vi "Periodic Tasks.vi"(8 "error in":errorcluster, 11 "RobotConfig":T17={"Motors"={"DriveLeftPrimary"={"CAN Address"=0, "Invert"=FALSE, "InvertSensor"=FALSE, "Unit Conversion Factor"=0.0, "Brake Mode"=enum."Override to Brake", "Reverse Limt Switch Mode"=enum."Normally Closed", "Forward Limt Swith Mode"=enum."Normally Closed", "PWM Channel"=enum."Invalid", "Motor Controller Type"=enum."Talon SRX"}, "DriveLeftSecondary1"={"CAN Address"=0, "Invert"=FALSE, "InvertSensor"=FALSE, "Unit Conversion Factor"=0.0, "Brake Mode"=enum."Override to Brake", "Reverse Limt Switch Mode"=enum."Normally Closed", "Forward Limt Swith Mode"=enum."Normally Closed", "PWM Channel"=enum."Invalid", "Motor Controller Type"=enum."Talon SRX"}, "DriveRightPrimary"={"CAN Address"=0, "Invert"=FALSE, "InvertSensor"=FALSE, "Unit Conversion Factor"=0.0, "Brake Mode"=enum."Override to Brake", "Reverse Limt Switch Mode"=enum."Normally Closed", "Forward Limt Swith Mode"=enum."Normally Closed", "PWM Channel"=enum."Invalid", "Motor Controller Type"=enum."Talon SRX"}, "DriveRightSecondary1"={"CAN Address"=0, "Invert"=FALSE, "InvertSensor"=FALSE, "Unit Conversion Factor"=0.0, "Brake Mode"=enum."Override to Brake", "Reverse Limt Switch Mode"=enum."Normally Closed", "Forward Limt Swith Mode"=enum."Normally Closed", "PWM Channel"=enum."Invalid", "Motor Controller Type"=enum."Talon SRX"}, "RightIntake"={"CAN Address"=8, "Invert"=FALSE, "InvertSensor"=FALSE, "Unit Conversion Factor"=0.0, "Brake Mode"=enum."Override to Brake", "Reverse Limt Switch Mode"=enum."Normally Closed", "Forward Limt Swith Mode"=enum."Normally Closed", "PWM Channel"=enum."Invalid", "Motor Controller Type"=enum."Talon SRX"}, "LeftIntake"={"CAN Address"=7, "Invert"=FALSE, "InvertSensor"=FALSE, "Unit Conversion Factor"=0.0, "Brake Mode"=enum."Override to Brake", "Reverse Limt Switch Mode"=enum."Normally Closed", "Forward Limt Swith Mode"=enum."Normally Closed", "PWM Channel"=enum."Invalid", "Motor Controller Type"=enum."Talon SRX"}, "ArmPivot"={"CAN Address"=5, "Invert"=FALSE, "InvertSensor"=FALSE, "Unit Conversion Factor"=0.0, "Brake Mode"=enum."Override to Brake", "Reverse Limt Switch Mode"=enum."Normally Closed", "Forward Limt Swith Mode"=enum."Normally Closed", "PWM Channel"=enum."Invalid", "Motor Controller Type"=enum."Talon SRX"}, "ArmExtend"={"CAN Address"=6, "Invert"=FALSE, "InvertSensor"=FALSE, "Unit Conversion Factor"=0.0, "Brake Mode"=enum."Override to Brake", "Reverse Limt Switch Mode"=enum."Normally Closed", "Forward Limt Swith Mode"=enum."Normally Closed", "PWM Channel"=enum."Invalid", "Motor Controller Type"=enum."Talon SRX"}, "ArmPivot2"={"CAN Address"=9, "Invert"=FALSE, "InvertSensor"=FALSE, "Unit Conversion Factor"=0.0, "Brake Mode"=enum."Override to Brake", "Reverse Limt Switch Mode"=enum."Normally Closed", "Forward Limt Swith Mode"=enum."Normally Closed", "PWM Channel"=enum."Invalid", "Motor Controller Type"=enum."Talon SRX"}, "Climber"={"CAN Address"=10, "Invert"=FALSE, "InvertSensor"=FALSE, "Unit Conversion Factor"=0.0, "Brake Mode"=enum."Override to Brake", "Reverse Limt Switch Mode"=enum."Disabled", "Forward Limt Swith Mode"=enum."Disabled", "PWM Channel"=enum."Invalid", "Motor Controller Type"=enum."Talon SRX"}, "Selfie Stick"={"CAN Address"=11, "Invert"=FALSE, "InvertSensor"=FALSE, "Unit Conversion Factor"=0.0, "Brake Mode"=enum."Override to Brake", "Reverse Limt Switch Mode"=enum."Disabled", "Forward Limt Swith Mode"=enum."Disabled", "PWM Channel"=enum."Invalid", "Motor Controller Type"=enum."Talon SRX"}}, "Sensors"={"IMU"={"Yaw Axis"=enum."X", "SPI Bus"=enum."SPI MXP", "AHRS Algorithm"=enum."Complementary", "Calibration Time (s)"=3.0, "Calibrate On Open"=FALSE}, "LimitSwitch1"={"DIOChannel"=enum."DIO 0", "Active Low"=FALSE}, "LimitSwitch2"={"DIOChannel"=enum."DIO 1", "Active Low"=FALSE}, "BeamBreak"={"DIOChannel"=enum."DIO 2", "Active Low"=FALSE}, "JeVois"={"Baud Rate"=9600, "Parity"=0, "Data Bits"=8, "Stop Bits"=10, "Termination Char (0xA = '\\n' = LF)"=10, "Enable Termination Char? (T)"=TRUE, "Flow Control"=0, "Timeout Value (ms)"=5000, "Serial Port"=enum."Onboard RS-232"}}, "PID"={"ArmExtend"={"P"=0.0, "I"=0.0, "D"=0.0, "F"=0.0, "IZone"=0.0}, "ArmRotate"={"P"=0.0, "I"=0.0, "D"=0.0, "F"=0.0, "IZone"=0.0}, "Drive"={"P"=0.0, "I"=0.0, "D"=0.0, "F"=0.0, "IZone"=0.0}, "DriveGyro Kp ((in/sec)/deg)"=0.0, "CameraPole"={"P"=0.0, "I"=0.0, "D"=0.0, "F"=0.0, "IZone"=0.0}}, "Solenoids"={"ArmClaw"={"Forward Channel"=enum."Solenoid 0", "Invert"=FALSE, "Reverse Channel"=enum."Solenoid 0"}, "IntakeExtend"={"Forward Channel"=enum."Solenoid 1", "Invert"=FALSE, "Reverse Channel"=enum."Solenoid 0"}, "IntakeOpen"={"Forward Channel"=enum."Solenoid 2", "Invert"=FALSE, "Reverse Channel"=enum."Solenoid 0"}, " Shifter"={"Forward Channel"=enum."Solenoid 3", "Invert"=FALSE, "Reverse Channel"=enum."Solenoid 0"}}, "RobotDimensions "={"Length"=0.0, "Height"=0.0, "HeightOfBumpers"=0.0, "DistanceFromFrameEdgeToPyramid "=0.0, "HeightOfFrameToIntake"=0.0, "EdgeOfFrameToOrigin"=0.0}, "ArmHomePosition"={"Angle (rad)"=0.0, "Radius (in)"=0.0}, "SelfieStickParams"={"Home Height (in)"=0.0, "CruiseVelocity"=0, "MaxAccel"=0, "Low Height (in)"=0.0, "High Height (in)"=0.0, "Mid Height (in)"=0.0}, "Enable Compressor"=TRUE} {"Sensors"."JeVois"."Flow Control" items=["None", "XON/XOFF", "RTS/CTS", "XON/XOFF & RTS/CTS", "DTR/DSR", "XON/XOFF & DTR/DSR"]; "Sensors"."JeVois"."Termination Char (0xA = '\\n' = LF)" format="%.0x"; "Sensors"."JeVois"."Stop Bits" items=["1.0"=10, "1.5"=15, "2.0"=20]; "Sensors"."JeVois"."Parity" items=["None", "Odd", "Even", "Mark", "Space"]}) -> ()   [LabVIEW 2017]
doc: "This VI runs in parallel to other tasks. It can contain as many user-defined periodic loops as you need. These can carry out PID or other sorts of timed response."
uses:
  PowerUpSrc/TypeDefs/ConfigComponents/Config_Robot.ctl
  ArgosLib/Config/ConfigComponents/TypeDefs/Config_Motor.ctl
  <vilib>/Rock Robotics/WPI/ThirdParty/Phoenix-LabVIEW/Motor Controller/Controls/CTRE_Phoenix_MotorControl_NeutralMode.ctl
  <vilib>/Rock Robotics/WPI/ThirdParty/Phoenix-LabVIEW/Motor Controller/Controls/CTRE_Phoenix_MotorControl_LimitSwitchNormal.ctl
  <vilib>/Rock Robotics/SystemInterfaces/DIO/FPGA_DIOPWMChannel.ctl
  ArgosLib/Config/ConfigComponents/TypeDefs/Config_MotorCtrlType.ctl
  ArgosLib/Config/ConfigComponents/TypeDefs/Config_IMU.ctl
  <vilib>/Rock Robotics/SystemInterfaces/spilib/spi_bus.ctl
  ArgosLib/Config/ConfigComponents/TypeDefs/Config_DigitalIO.ctl
  <vilib>/Rock Robotics/SystemInterfaces/DIO/FPGA_DIOChannel.ctl
  ArgosLib/Config/ConfigComponents/TypeDefs/Config_SerialPort.ctl
  <vilib>/Rock Robotics/WPI/SerialPort/WPI_SerialPort.ctl
  ArgosLib/Config/ConfigComponents/TypeDefs/Config_PIDParams.ctl
  ArgosLib/Config/ConfigComponents/TypeDefs/Config_DoubleSolenoid.ctl
  <vilib>/Rock Robotics/WPI/Solenoid/WPI_SolenoidChannel.ctl
  PowerUpSrc/TypeDefs/ConfigComponents/Config_Dimensions.ctl
  PowerUpSrc/TypeDefs/ConfigComponents/Config_ArmHome.ctl
  PowerUpSrc/TypeDefs/ConfigComponents/Config_SelfieStick.ctl
  ArgosLib/Miscellaneous/TypeDefs/ArgoDriveJoystickMap.ctl
  ArgosLib/Miscellaneous/TypeDefs/LookUpTableParameters.ctl
  PowerUpSrc/Implements/Arm/TypeDefs/ArmPositions.ctl
  ArgosLib/Path Planning/TypeDefs/Point2D.ctl
  PowerUpSrc/General/MotionProfiling/TypeDefs/MotionProfileGeneratorParams.ctl
  <vilib>/Rock Robotics/WPI/ThirdParty/Phoenix-LabVIEW/Motor Controller/Controls/CTRE_Phoenix_MotorControl_TrajectoryPointTimeDur.ctl
  PowerUpSrc/Autonomous/PathPlannerSupport/TypeDefs/DrivePathfinderParams.ctl
  PowerUpSrc/Autonomous/TypeDef/AutoStep.ctl
  PowerUpSrc/Autonomous/TypeDef/AutoWaypointType.ctl
  Pathfinder/Pathfinder-LabVIEW/Pathfinder-Lib/VIs/Waypoint.ctl
  PowerUpSrc/Implements/Arm/TypeDefs/ArmTargetPosition.ctl
  PowerUpSrc/Implements/TypeDefs/IntakeState.ctl
  PowerUpSrc/Autonomous/TypeDef/AutoStartingPositions.ctl
  PowerUpSrc/Autonomous/TypeDef/AutoFieldState.ctl
  <vilib>/Rock Robotics/WPI/DriverStation/WPI_DriverStationRobotMode2.ctl
  ArgosLib/Signal Processing/TypeDefs/EdgeDetector_Type.ctl
  <vilib>/Rock Robotics/WPI/Solenoid/WPI_SolenoidValue.ctl
  PowerUpSrc/Implements/Arm/TypeDefs/ArmHomingState.ctl
  PowerUpSrc/General/MotionProfiling/TypeDefs/MotionProfileControlState.ctl
  <vilib>/Rock Robotics/WPI/ThirdParty/Phoenix-LabVIEW/Motor Controller/Controls/CTRE_Phoenix_MotorControl_ControlMode.ctl
  <vilib>/Rock Robotics/WPI/Utilities/WPI_GetSetVariantRefNum.vi
  PowerUpSrc/Global_Var-RefNum/LEDData.vi
  PowerUpSrc/Global_Var-RefNum/Joystick_Control.vi
  <vilib>/Rock Robotics/WPI/Solenoid/WPI_SolenoidSetEnum.vi
  PowerUpSrc/Global_Var-RefNum/SwitchedCameraData.vi
  ArgosLib/ArgosLib.lvlib
  PowerUpSrc/Sensors/IMU/ADIS16448_IMU.lvlib
  69abced5-d8d5-48e2-b3a2-692bc54adc8e.vi
  Pathfinder/Pathfinder-LabVIEW/Pathfinder-Lib/Pathfinder.lvlib
panel:
  out "ActiveTestRoutine":string
  in  "AutoTest":bool
  out "AutoControl":bool
  out "ArmReadyForAuto":bool
  out "LED Loop Rate (Hz)":dbl
  in  "Reload Routines":bool
  in  "Auto Routines Storage Directory":path=path "/home/lvuser/AutoRoutines"
  in  "Auto Routine":u16(ring) items=["Auto Line", "Auto Line (Reverse)", "Left Switch->Left Scale", "Left Switch->Left Switch->Left Scale", "Left Switch->Left Switch", "Left Switch->Left Switch (Back)", "Left Switch->Right Scale", "Left Switch", "Right Switch->Left Scale", "Right Switch->Right Scale", "Right Switch->Right Switch->Right Scale", "Right Switch->Right Switch", "Right Switch->Right Switch (Back)", "Right Switch"]
  in  "AutoStartingPosition":T1
  in  "CustomAutoSteps":bool
  in  "AutoInTeleop":bool
  in  "AutoStart":bool
  out "AutoIntakeState":T2
  out "AutoClawOpen":bool
  in  "AutoSteps":T3[](array[typedef])=[{"Waypoint Type"=enum."Pathfinder Endpoint", "Waypoint"={"x"=19.5, "y"=50.0, "angle"=0.0}, "WaitTime (ms)"=0, "ArmPosition"=enum."Hold", "IntakeState"=enum."Stop", "Claw Open"=FALSE, "ArmOffsetTime (ms)"=0, "ClawReleaseTime (ms)"=0}, {"Waypoint Type"=enum."Pathfinder Waypoint", "Waypoint"={"x"=180.0, "y"=50.0, "angle"=0.0}, "WaitTime (ms)"=0, "ArmPosition"=enum."Hold", "IntakeState"=enum."Stop", "Claw Open"=FALSE, "ArmOffsetTime (ms)"=0, "ClawReleaseTime (ms)"=0}, {"Waypoint Type"=enum."Pathfinder Waypoint", "Waypoint"={"x"=270.0, "y"=135.0, "angle"=90.0}, "WaitTime (ms)"=0, "ArmPosition"=enum."Hold", "IntakeState"=enum."Stop", "Claw Open"=FALSE, "ArmOffsetTime (ms)"=0, "ClawReleaseTime (ms)"=0}, {"Waypoint Type"=enum."Pathfinder Waypoint", "Waypoint"={"x"=270.0, "y"=260.0, "angle"=90.0}, "WaitTime (ms)"=0, "ArmPosition"=enum."Hold", "IntakeState"=enum."Stop", "Claw Open"=FALSE, "ArmOffsetTime (ms)"=0, "ClawReleaseTime (ms)"=0}, {"Waypoint Type"=enum."Pathfinder Endpoint", "Waypoint"={"x"=180.0, "y"=350.0, "angle"=180.0}, "WaitTime (ms)"=0, "ArmPosition"=enum."Hold", "IntakeState"=enum."Stop", "Claw Open"=FALSE, "ArmOffsetTime (ms)"=0, "ClawReleaseTime (ms)"=0}, {"Waypoint Type"=enum."Zero-Radius Turn Endpoint", "Waypoint"={"x"=0.0, "y"=0.0, "angle"=180.0}, "WaitTime (ms)"=0, "ArmPosition"=enum."Hold", "IntakeState"=enum."Stop", "Claw Open"=FALSE, "ArmOffsetTime (ms)"=0, "ClawReleaseTime (ms)"=0}, {"Waypoint Type"=enum."Zero-Radius Turn Endpoint", "Waypoint"={"x"=0.0, "y"=0.0, "angle"=290.0}, "WaitTime (ms)"=0, "ArmPosition"=enum."Switch", "IntakeState"=enum."Stop", "Claw Open"=FALSE, "ArmOffsetTime (ms)"=0, "ClawReleaseTime (ms)"=0}, {"Waypoint Type"=enum."Pathfinder Endpoint", "Waypoint"={"x"=180.0, "y"=320.0, "angle"=270.0}, "WaitTime (ms)"=0, "ArmPosition"=enum."Switch", "IntakeState"=enum."Stop", "Claw Open"=FALSE, "ArmOffsetTime (ms)"=0, "ClawReleaseTime (ms)"=0}, {"Waypoint Type"=enum."Pathfinder Endpoint", "Waypoint"={"x"=180.0, "y"=300.0, "angle"=270.0}, "WaitTime (ms)"=0, "ArmPosition"=enum."Switch", "IntakeState"=enum."Stop", "Claw Open"=FALSE, "ArmOffsetTime (ms)"=0, "ClawReleaseTime (ms)"=0}, {"Waypoint Type"=enum."Stationary", "Waypoint"={"x"=0.0, "y"=0.0, "angle"=0.0}, "WaitTime (ms)"=250, "ArmPosition"=enum."Hold", "IntakeState"=enum."Stop", "Claw Open"=TRUE, "ArmOffsetTime (ms)"=0, "ClawReleaseTime (ms)"=0}]
  out "Auto Loop Rate (Hz)":dbl
  in  "DrivePathPlanParams":T7={"max_velocity (in/s)"=70.0, "max_acceleration (in/s^2)"=200.0, "max_jerk (in/s^3)"=300.0, "dt(ms)"=40, "sample_count"=1000, "wheelbase_width (in)"=25.0} {"dt(ms)" items=["TrajectoryDuration_0ms"=0, "TrajectoryDuration_5ms"=5, "TrajectoryDuration_10ms"=10, "TrajectoryDuration_20ms"=20, "TrajectoryDuration_30ms"=30, "TrajectoryDuration_40ms"=40, "TrajectoryDuration_50ms"=50, "TrajectoryDuration_100ms"=100]}
  in  "DriveGyro Kp ((in/sec)/deg)":dbl=-0.5
  in  "Turning_Still_Multiplier":dbl=2.5
  out "IMU Angles Out":T9
  out "Drive Velocity Loop Rate (Hz)":dbl
  out "Arm Planner Loop Rate (Hz)":dbl
  out "Drive Planner Loop Rate (Hz)":dbl
  out "MP Loop Rate (Hz)":dbl
  out "Implement Loop Rate (Hz)":dbl
  out "JeVois Loop Rate (Hz)":dbl
  out "Compressor Loop Rate (Hz)":dbl
  out "Drive Loop Rate (Hz)":dbl
  in  "DriveControlMode":enum16{"Tuning", "TestPathPlanner", "Auto"}(ring)=enum."Auto"
  in  "ClimbSpeed":dbl=1.0 format="%#_13g"
  out "ArmExtendMapping":T10(graph)
  out "ArmPivotMapping":T10(graph)
  in  "ArmExtendControlsMap":T11={"Look Up Table OUT"=[-0.5, 0.0, 0.0, 0.5], "Look Up Table IN"=[-1.0, -0.2, 0.2, 1.0]}
  in  "ArmPivotControlsMap":T11={"Look Up Table OUT"=[-0.6, 0.0, 0.0, 0.6], "Look Up Table IN"=[-1.0, -0.2, 0.2, 1.0]}
  in  "ArmMotionProfileGeneratorParameters":T12={"Trajectory Point Interval (ms)"=40, "Maximum Travel Speed (units/s)"=110.0, "Velocity Ramp Time (ms)"=200.0, "Acceleration Ramp Time (ms)"=100.0} {"Acceleration Ramp Time (ms)" min=1.0; "Velocity Ramp Time (ms)" min=1.0; "Maximum Travel Speed (units/s)" min=0.0; "Trajectory Point Interval (ms)" items=["TrajectoryDuration_0ms"=0, "TrajectoryDuration_5ms"=5, "TrajectoryDuration_10ms"=10, "TrajectoryDuration_20ms"=20, "TrajectoryDuration_30ms"=30, "TrajectoryDuration_40ms"=40, "TrajectoryDuration_50ms"=50, "TrajectoryDuration_100ms"=100]}
  in  "Arm max Extension (in)":dbl=68.0
  in  "Arm min Extension (in)":dbl=44.0
  in  "Arm positions":T13={"Hold"={"X"=22.4, "Y"=-39.5}, "High Scale"={"X"=40.0, "Y"=48.959}, "Low Scale"={"X"=40.0, "Y"=22.496}, "Switch"={"X"=43.0, "Y"=-9.338}, "Climb"={"X"=6.323, "Y"=48.113}, "Back Place"={"X"=-12.0, "Y"=48.0}}
  in  "ArmControlMode":enum16{"Tuning", "TestPathPlanner", "Operator"}(ring)=enum."Operator"
  in  "Intake_Speed":dbl=1.0
  in  "Argo Drive Joystick Map":T15={"Auto Speed"={"Look Up Table OUT"=[-1.0, -0.75, -0.06, -0.05, 0.0, 0.05, 0.06, 0.75, 1.0], "Look Up Table IN"=[-1.0, -0.75, -0.06, -0.05, 0.0, 0.05, 0.06, 0.75, 1.0]}, "Low Speed"={"Look Up Table OUT"=[-1.0, -0.4, -0.15, 0.0, 0.0, 0.0, 0.15, 0.4, 1.0], "Look Up Table IN"=[-1.0, -0.75, -0.21, -0.2, 0.0, 0.2, 0.21, 0.75, 1.0]}, "Auto Turning"={"Look Up Table OUT"=[-1.0, -0.75, -0.12, -0.1, 0.0, 0.1, 0.12, 0.75, 1.0], "Look Up Table IN"=[-1.0, -0.75, -0.12, -0.1, 0.0, 0.1, 0.12, 0.75, 1.0]}, "Low Turning"={"Look Up Table OUT"=[-0.4, -0.2, 0.0, 0.0, 0.0, 0.0, 0.2, 0.4], "Look Up Table IN"=[-1.0, -0.75, -0.2, -0.19, 0.19, 0.2, 0.75, 1.0]}, "High Speed"={"Look Up Table OUT"=[-0.8, -0.5, -0.15, 0.0, 0.0, 0.0, 0.15, 0.5, 0.8], "Look Up Table IN"=[-1.0, -0.75, -0.16, -0.15, 0.0, 0.15, 0.16, 0.75, 1.0]}, "High Turning"={"Look Up Table OUT"=[-0.15, 0.0, 0.0, 0.0, 0.15], "Look Up Table IN"=[-1.0, -0.2, 0.0, 0.2, 1.0]}}
  out "Encoder Outputs":T16
  in  "WheelDiameter(in)":dbl=4.0
  in  "CountsPerRevolution":i32=4096
  in  "ZeroEncoders":bool
  # "Loop Rates"
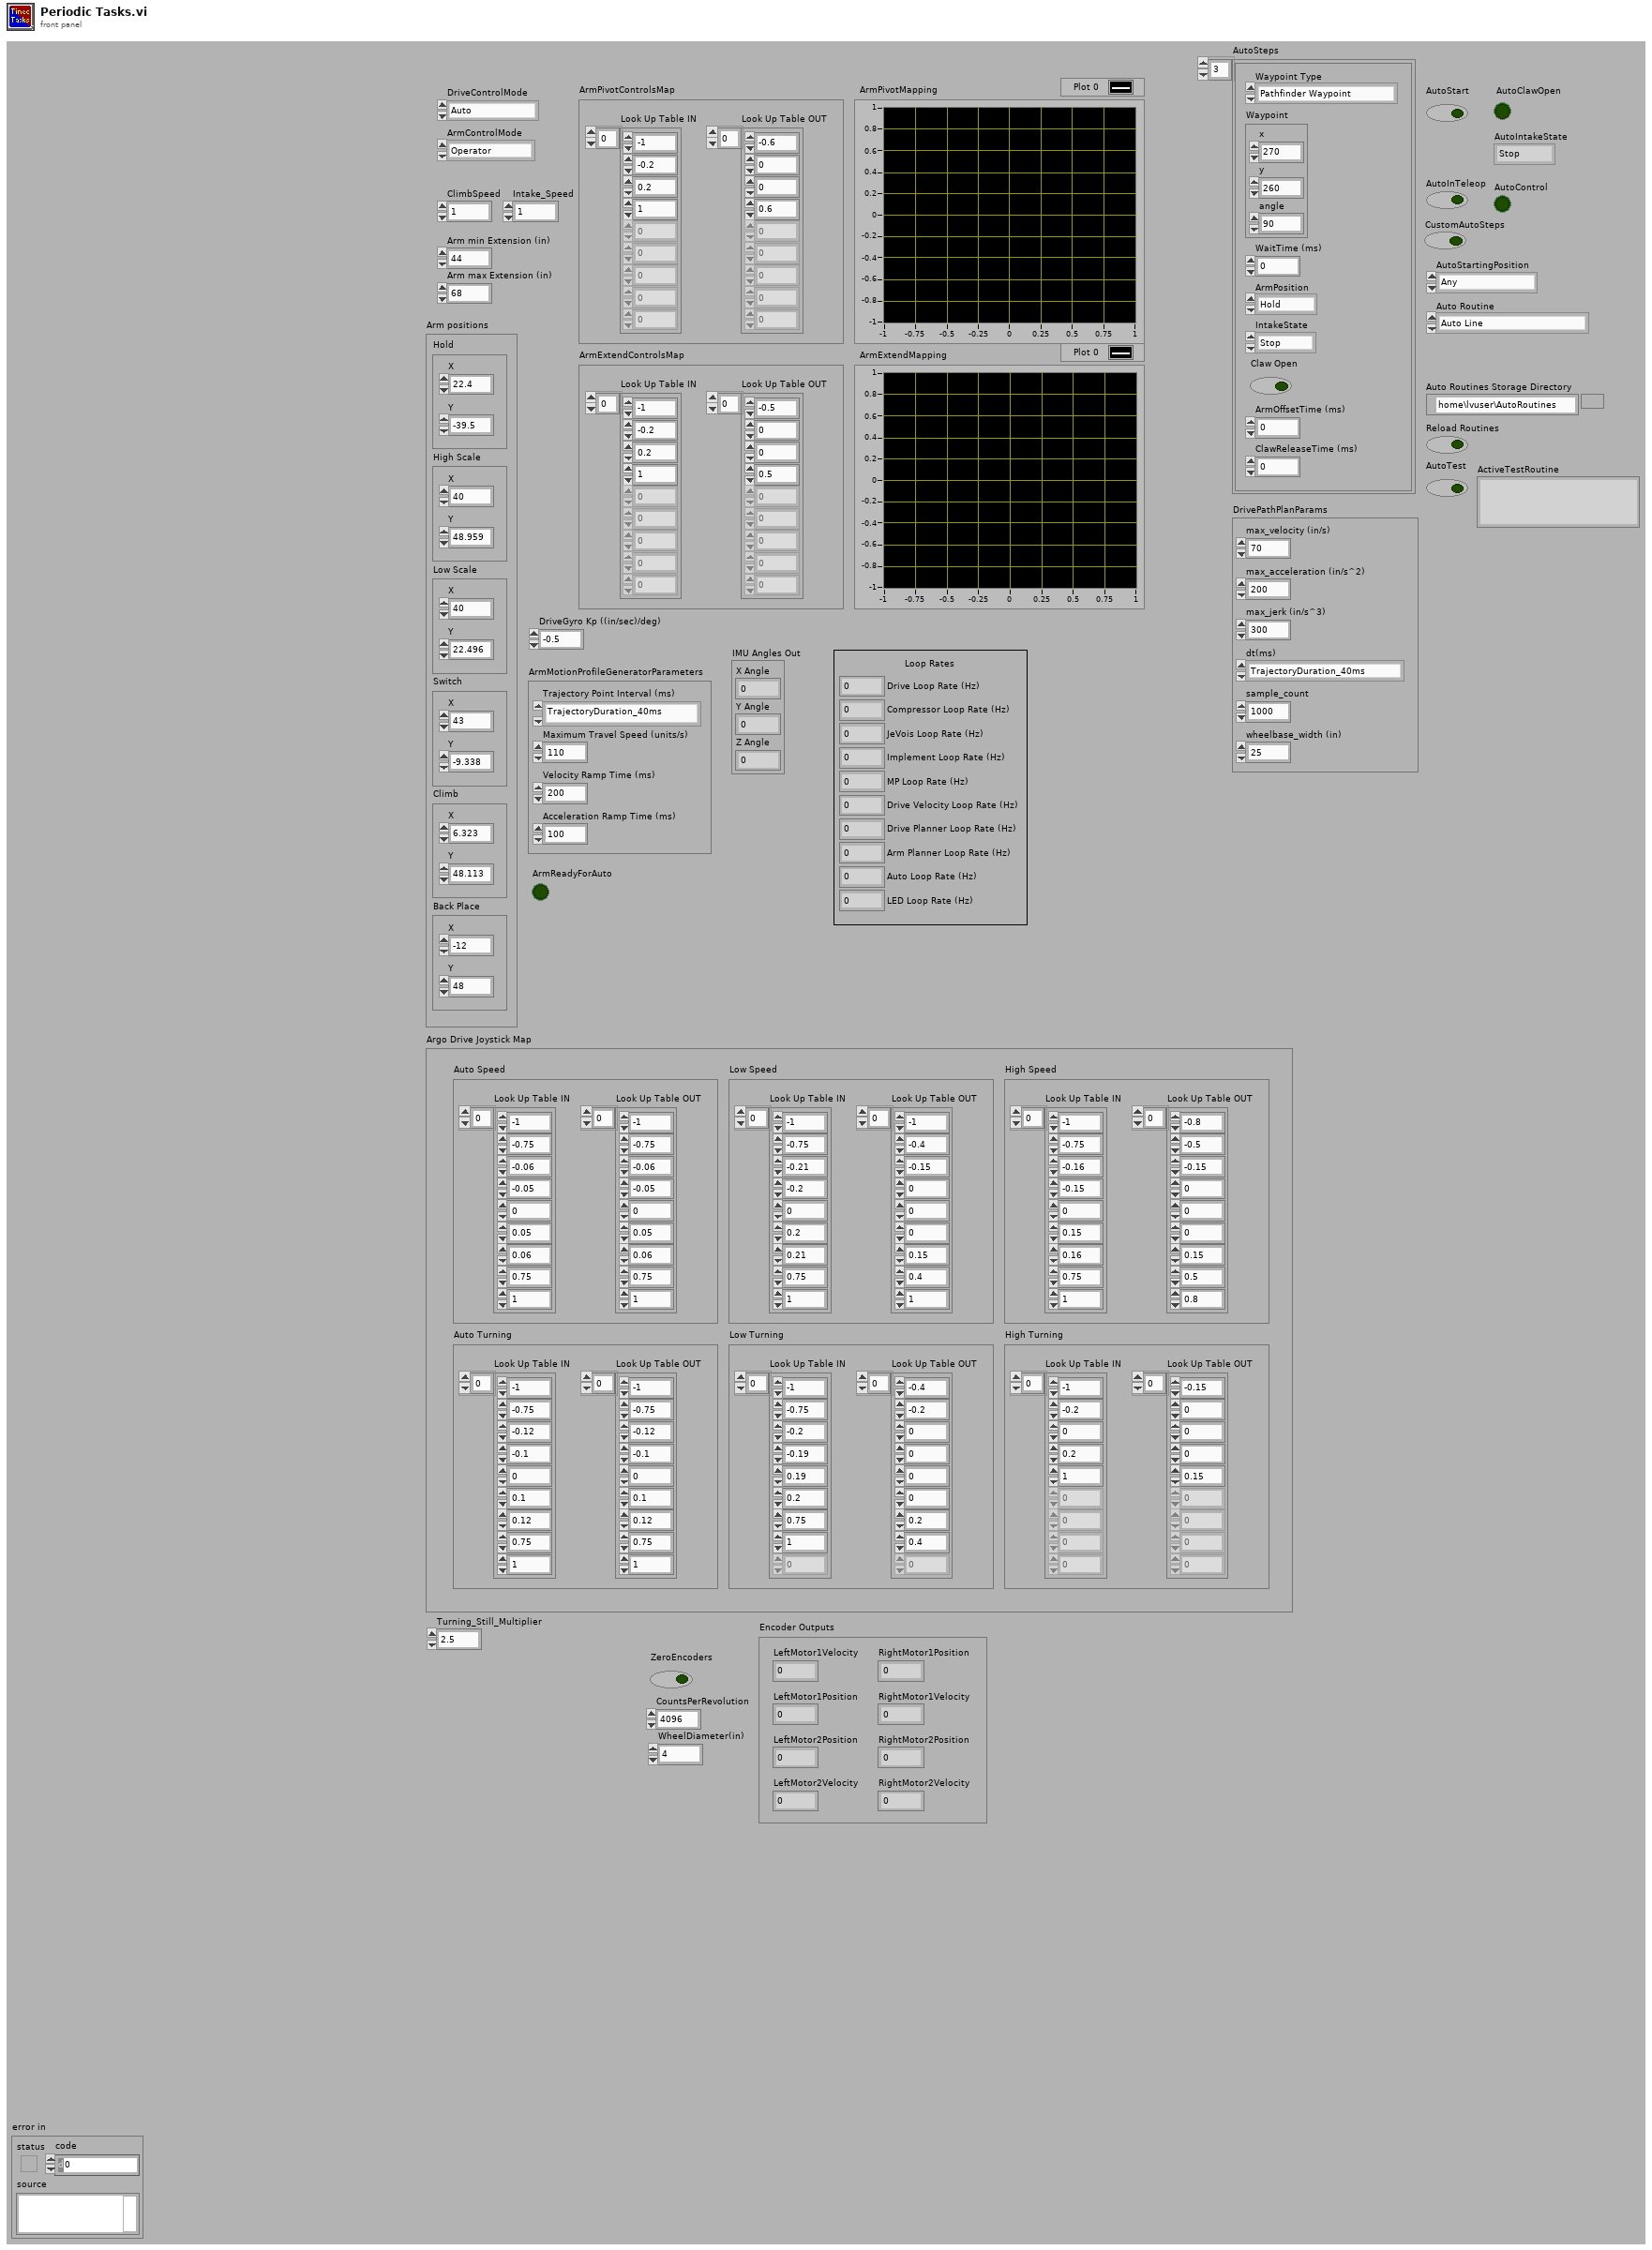
[diagram p1: front panel]
types:
  T1 = typedef "AutoStartingPositions.ctl" = enum16{"Any", "Left", "Center", "Right"}
  T2 = typedef "IntakeState.ctl" = enum16{"Stop", "Forward", "Reverse", "Forward Open"}
  T3 = typedef "AutoStep.ctl" = cluster{"Waypoint Type":T4, "Waypoint":T5, "WaitTime (ms)":u16, "ArmPosition":T6, "IntakeState":T2, "Claw Open":bool, "ArmOffsetTime (ms)":u16, "ClawReleaseTime (ms)":i32}
  T4 = typedef "AutoWaypointType.ctl" = enum16{"Pathfinder Endpoint", "Pathfinder Waypoint", "Zero-Radius Turn Endpoint", "Stationary", "Vision Assist Endpoint", "Stop"}
  T5 = typedef "Pathfinder.lvlib/Waypoint.ctl" = cluster{"x":dbl, "y":dbl, "angle":dbl}
  T6 = typedef "ArmTargetPosition.ctl" = enum16{"Hold", "Switch", "Scale Low", "Scale High", "Climb", "Back Place"}
  T7 = typedef "DrivePathfinderParams.ctl" = cluster{"max_velocity (in/s)":dbl, "max_acceleration (in/s^2)":dbl, "max_jerk (in/s^3)":dbl, "dt(ms)":T8, "sample_count":i32, "wheelbase_width (in)":dbl}
  T8 = typedef "CTRE_Phoenix_MotorControl_TrajectoryPointTimeDur.ctl" = i32
  T9 = cluster{"X Angle":dbl, "Y Angle":dbl, "Z Angle":dbl}
  T10 = cluster{"Look Up Table OUT":dbl[], "Look Up Table IN":dbl[]}
  T11 = typedef "ArgosLib.lvlib/LookUpTableParameters.ctl" = cluster{"Look Up Table OUT":dbl[], "Look Up Table IN":dbl[]}
  T12 = typedef "MotionProfileGeneratorParams.ctl" = cluster{"Trajectory Point Interval (ms)":T8, "Maximum Travel Speed (units/s)":dbl, "Velocity Ramp Time (ms)":dbl, "Acceleration Ramp Time (ms)":dbl}
  T13 = typedef "ArmPositions.ctl" = cluster{"Hold":T14, "High Scale":T14, "Low Scale":T14, "Switch":T14, "Climb":T14, "Back Place":T14}
  T14 = typedef "Point2D.ctl" = cluster{"X":dbl, "Y":dbl}
  T15 = typedef "ArgosLib.lvlib/ArgoDriveJoystickMap.ctl" = cluster{"Auto Speed":T11, "Low Speed":T11, "Auto Turning":T11, "Low Turning":T11, "High Speed":T11, "High Turning":T11}
  T16 = cluster{"LeftMotor1Velocity ":dbl, "LeftMotor1Position":dbl, "RightMotor1Velocity ":dbl, "RightMotor1Position ":dbl, "LeftMotor2Position ":dbl, "LeftMotor2Velocity ":dbl, "RightMotor2Position":dbl, "RightMotor2Velocity":dbl}
  T17 = typedef "Config_Robot.ctl" = cluster{"Motors":cluster{"DriveLeftPrimary":T18, "DriveLeftSecondary1":T18, "DriveRightPrimary":T18, "DriveRightSecondary1":T18, "RightIntake":T18, "LeftIntake":T18, "ArmPivot":T18, "ArmExtend":T18, "ArmPivot2":T18, "Climber":T18, "Selfie Stick":T18}, "Sensors":cluster{"IMU":T23, "LimitSwitch1":T25, "LimitSwitch2":T25, "BeamBreak":T25, "JeVois":T27}, "PID":cluster{"ArmExtend":T29, "ArmRotate":T29, "Drive":T29, "DriveGyro Kp ((in/sec)/deg)":dbl, "CameraPole":T29}, "Solenoids":cluster{"ArmClaw":T30, "IntakeExtend":T30, "IntakeOpen":T30, " Shifter":T30}, "RobotDimensions ":T32, "ArmHomePosition":T33, "SelfieStickParams":T34, "Enable Compressor":bool}
  T18 = typedef "Config_Motor.ctl" = cluster{"CAN Address":u8, "Invert":bool, "InvertSensor":bool, "Unit Conversion Factor":dbl, "Brake Mode":T19, "Reverse Limt Switch Mode":T20, "Forward Limt Swith Mode":T20, "PWM Channel":T21, "Motor Controller Type":T22}
  T19 = typedef "CTRE_Phoenix_MotorControl_NeutralMode.ctl" = enum8{"EEPROMSetting", "Override to Coast", "Override to Brake"}
  T20 = typedef "CTRE_Phoenix_MotorControl_LimitSwitchNormal.ctl" = enum16{"Normally Open", "Normally Closed", "Disabled"}
  T21 = typedef "FPGA_DIOPWMChannel.ctl" = enum8{"PWM 0", "PWM 1", "PWM 2", "PWM 3", "PWM 4", "PWM 5", "PWM 6", "PWM 7", "PWM 8", "PWM 9", "PWM MXP 0", "PWM MXP 1", "PWM MXP 2", "PWM MXP 3", "PWM MXP 4", "PWM MXP 5", "PWM MXP 6", "PWM MXP 7", "PWM MXP 8", "PWM MXP 9", "Invalid"}
  T22 = typedef "Config_MotorCtrlType.ctl" = enum16{"Disabled", "Talon SRX", "Talon SR"}
  T23 = typedef "Config_IMU.ctl" = cluster{"Yaw Axis":enum16{"X", "Y", "Z"}, "SPI Bus":T24, "AHRS Algorithm":enum16{"Complementary", "Madgwick"}, "Calibration Time (s)":dbl, "Calibrate On Open":bool}
  T24 = typedef "spi_bus.ctl" = enum16{"SPI On-Board, CS0", "SPI On-Board, CS1", "SPI On-Board, CS2", "SPI On-Board, CS3", "SPI MXP", "Invalid"}
  T25 = typedef "Config_DigitalIO.ctl" = cluster{"DIOChannel":T26, "Active Low":bool}
  T26 = typedef "FPGA_DIOChannel.ctl" = enum8{"DIO 0", "DIO 1", "DIO 2", "DIO 3", "DIO 4", "DIO 5", "DIO 6", "DIO 7", "DIO 8", "DIO 9", "DIO MXP 0", "DIO MXP 1", "DIO MXP 2", "DIO MXP 3", "DIO MXP 4", "DIO MXP 5", "DIO MXP 6", "DIO MXP 7", "DIO MXP 8", "DIO MXP 9", "DIO MXP 10", "DIO MXP 11", "DIO MXP 12", "DIO MXP 13", "DIO MXP 14", "DIO MXP 15", "SPI Port CS1", "SPI Port CS2", "SPI Port CS3", "SPI Port MISO", "SPI Port MOSI", "Invalid"}
  T27 = typedef "Config_SerialPort.ctl" = cluster{"Baud Rate":u32, "Parity":u16, "Data Bits":u16, "Stop Bits":u16, "Termination Char (0xA = '\\n' = LF)":u8, "Enable Termination Char? (T)":bool, "Flow Control":u16, "Timeout Value (ms)":u32, "Serial Port":T28}
  T28 = typedef "WPI_SerialPort.ctl" = enum16{"Onboard RS-232", "MXP TTL", "USB 1", "USB 2"}
  T29 = typedef "Config_PIDParams.ctl" = cluster{"P":dbl, "I":dbl, "D":dbl, "F":dbl, "IZone":dbl}
  T30 = typedef "Config_DoubleSolenoid.ctl" = cluster{"Forward Channel":T31, "Invert":bool, "Reverse Channel":T31}
  T31 = typedef "WPI_SolenoidChannel.ctl" = enum8{"Solenoid 0", "Solenoid 1", "Solenoid 2", "Solenoid 3", "Solenoid 4", "Solenoid 5", "Solenoid 6", "Solenoid 7", "Invalid"}
  T32 = typedef "Config_Dimensions.ctl" = cluster{"Length":dbl, "Height":dbl, "HeightOfBumpers":dbl, "DistanceFromFrameEdgeToPyramid ":dbl, "HeightOfFrameToIntake":dbl, "EdgeOfFrameToOrigin":dbl}
  T33 = typedef "Config_ArmHome.ctl" = cluster{"Angle (rad)":dbl, "Radius (in)":dbl}
  T34 = typedef "Config_SelfieStick.ctl" = cluster{"Home Height (in)":dbl, "CruiseVelocity":i32, "MaxAccel":i32, "Low Height (in)":dbl, "High Height (in)":dbl, "Mid Height (in)":dbl}
  T35 = typedef "RobotJoysticks.ctl" = cluster{"Driver Controller":T36, "Operator Controller":T36}
  T36 = typedef "WPI_JoystickDevRef.ctl" = cluster{"Device":T37}
  T37 = typedef "WPI_JoystickDeviceEnum.ctl" = enum16{"USB 0", "USB 1", "USB 2", "USB 3", "USB 4", "USB 5"}
  T38 = typedef "WPI_RobotDriveDevRef.ctl" = cluster{"DevStatus":errorcluster, "Motors[]":T39[], "Square Inputs":bool, "Max Output":dbl}
  T39 = typedef "WPI_MotorControlDeviceRef.ctl" = cluster{"DeviceStatus":errorcluster, "Type":T40, "PWM":cluster{"PWM Channel":T21, "DeadBand":T41}, "CAN":cluster{"Device Number":u8, "SetOutput VI Ref":variant, "GetOutput VI Ref":variant, "Enable VI Ref":variant, "Disable VI Ref":variant, "Data":variant}, "Invert":bool, "DIO PWM":cluster{"PWM \"Enable\" Channel":T21, "DIOChannel":T26, "PWM Rate":dbl}}
  T40 = typedef "WPI_MotorControlType.ctl" = enum16{"PWM", "CAN", "DIO PWM"}
  T41 = typedef "WPI_PWMDeadband.ctl" = cluster{"Name":string, "maxPositivePwm":i32, "minPositivePwm":i32, "centerPwm":i32, "maxNegativePwm":i32, "minNegativePwm":i32, "angularRange":u16}
  T42 = typedef "RobotMotors.ctl" = cluster{"DriveLeftPrimary":T39, "DriveLeftSecondary1":T39, "DriveRightPrimary":T39, "DriveRightSecondary1":T39, " RightIntake":T39, "LeftIntake":T39, "ArmPivot":T39, "ArmPivot 2 ":T39, "ArmExtend ":T39, "Climber":T39, "SelfieStick":T39}
  T43 = typedef "RobotPneumatics.ctl" = cluster{"ArmClaw":T44, "IntakeExtend":T44, "IntakeOpen":T44, "Shifter":T44, "Compressor":T45}
  T44 = typedef "WPI_SolenoidDevRef.ctl" = cluster{"DevStatus":errorcluster, "Pneumatics Control Module":u8, "Forward Solenoid Channel":T31, "Reverse Solenoid Channel":T31}
  T45 = typedef "WPI_CompressorDevRef.ctl" = cluster{"DevStatus":errorcluster, "Pneumatics Control Module":u8}
  T46 = typedef "RobotSensors.ctl" = cluster{"IMU":T47, "BeamBreak":T48, "JeVois":T49}
  T47 = typedef "ADIS16448_IMU.lvlib/ADI_IMU_ADIS16448_IMUDevRef.ctl" = cluster{"DevStatus":errorcluster, "Handle":i32, "SPI Bus":T24, "Device Found":bool, "Device Ready":bool, "Yaw Axis":enum16{"X", "Y", "Z"}, "AHRS Algorithm":enum16{"Complementary", "Madgwick"}, "Serial":u16, "Lot ID 2":u16, "Lot ID 1":u16, "Bytes Per Sample":u16, "Calibrate On Open?":bool}
  T48 = typedef "WPI_DigitalInputDevRef.ctl" = cluster{"DevStatus":errorcluster, "DIO Channel":T26}
  T49 = typedef "WPI_SerialPortRef.ctl" = cluster{"DevStatus":errorcluster, "Serial Port Name":refnum<visa-resource-name>}
  T50 = typedef "MotionPlanningNotifiers.ctl" = cluster{"DrivePlanRequestNotifier":refnum<notifier>, "DrivePlanResponseNotifier":refnum<notifier>, "ArmPlanRequestNotifier":refnum<notifier>, "ArmPlanResponseNotifier":refnum<notifier>, "DriveCompleteNotifier":refnum<notifier>, "ArmCompleteNotifier":refnum<notifier>}
  T51 = cluster{"RobotConfig":T17, "Joysticks":T35, "RobotDriveDevRef":T38, "RobotMotorsOut":T42, "Pneumatics":T43, "Sensors":T46, "MotionPlanningNotifiers":T50}
  T52 = typedef "WPI_SolenoidValue.ctl" = enum16{"Off", "On", "Forward", "Reverse"}
  T53 = typedef "JoystickControls.ctl" = cluster{"drive speed":dbl, "drive turning":dbl, "Unassigned_LX":dbl, "Unassigned_RY":dbl, "Cube Release":bool, "Intake Forward":dbl, "Intake Reverse ":dbl, "Switch":bool, "Scale Low":bool, "Scale High":bool, "Shift":bool, "Arm To Preset":bool, "Win_LJ":bool, "Win_RJ":bool, "Swap/ClimbPosition_Back":bool, "Swap_Start":bool, "Arm Extend/Retract":dbl, "Unassigned_RX 2":dbl, "Unassigned_LX 2":dbl, "Arm  Pivot Up/Down ":dbl, "Cube Release 2":bool, "Extend/Retract Intake":dbl, "Open/Close Intake":dbl, "Switch 2":bool, "Scale High 2":bool, "Scale Low 2":bool, "Claw Pinch 2":bool, "Arm Hold":bool, "Unassigned_LJ 2":bool, "Unassigned_RJ 2":bool, "Swap/ClimbPosition_Back 2":bool, "Swap/SelfieStick_Start 2":bool, "Climb Up 2":bool, "Unassigned_Right 2":bool, "Climb Down 2":bool, "Unassigned_Left 2":bool, "Climb Up ":bool, " Unassigned_Right":bool, "Climb Down":bool, "Unassigned_Left":bool}
  T54 = typedef "Pathfinder.lvlib/Segment.ctl" = cluster{"dt":dbl, "x":dbl, "y":dbl, "position":dbl, "velocity":dbl, "acceleration":dbl, "jerk":dbl, "heading":dbl}
  T55 = typedef "DrivePlanResponse.ctl" = cluster{"LeftDriveTrajectory":T54[], "RightDriveTrajectory":T54[], "PlanTime (ms)":u32, "Execute":bool}
  T56 = cluster{"LeftMotor1Position ":dbl, "LeftMotor1Velocity":dbl, "RightMotor1Velocity ":dbl, "RightMotor1Position ":dbl, "LeftMotor2Position ":dbl, "LeftMotor2Velocity ":dbl, "RightMotor2Position":dbl, "RightMotor2Velocity":dbl}
  T57 = cluster{"LeftMotor1Position ":i32, "LeftMotor1Velocity":i32, "RightMotor1Velocity ":i32, "RightMotor1Position ":i32, "LeftMotor2Position ":i32, "LeftMotor2Velocity ":i32, "RightMotor2Position":i32, "RightMotor2Velocity":i32}
  T58 = typedef "WPI_DriverStationRobotMode2.ctl" = enum16{"Autonomous Disabled", "Autonomous Enabled", "Teleop Disabled", "Teleop Enabled", "Disconnected", "Finish", "Test Disabled", "Test Enabled", "Emergency Stopped"}
  T59 = typedef "MotionProfileControlState.ctl" = enum16{"Manual", "Auto_Idle", "Auto_Run"}
  T60 = typedef "ArgosLib.lvlib/EdgeDetector_Type.ctl" = enum16{"RisingEdge", "FallingEdge", "Both"}
  T61 = typedef "ArmHomingState.ctl" = enum16{"ready", "go to home", "homing complete ", "homing failed"}
  T62 = typedef "Polygon2D.ctl" = T14[]
  T63 = typedef "TrajectoryPoint.ctl" = cluster{"Position ":dbl, "Velocity ":dbl, "Time (ms)":T8, "Last Point":bool}
  T64 = typedef "ArmPlanRequest.ctl" = cluster{"Destination":T6, "Preview":bool, "Start":T6, "Fixed Start":bool}
  T65 = typedef "ArmPlanResponse.ctl" = cluster{"RotateTrajectory":T63[], "ExtendTrajectory":T63[], "PlanTime (ms)":u32, "Execute":bool}
  T66 = cluster{"Look Up Table IN":dbl[], "Look Up Table OUT":dbl[]}
  T67 = typedef "CTRE_Phoenix_MotorControl_ControlMode.ctl" = u16
  T68 = typedef "DrivePlanRequest.ctl" = cluster{"Plan Type":T4, "Waypoints":T5[], "Preview":bool}
  T69 = typedef "AutoFieldState.ctl" = enum16{"Left-Left-Left", "Left-Right-Left", "Right-Left-Right", "Right-Right-Right", "Unknown"}
  T70 = typedef "Game_Data.ctl" = cluster{"Close  Switch":T71, "Scale":T71, "Far Switch":T71}
  T71 = typedef "Plate_Positions.ctl" = enum16{"Left", "Right", "Unknown"}
  T72 = typedef "AutoRoutineSet.ctl" = cluster{"Routine Names":string[], "Routines":path[]}
  T73 = typedef "AutoPreProcessedStep.ctl" = cluster{"DrivePath":T55, "ArmPath":T65, "Waypoint Type":T4, "WaitTime (ms)":u16, "ArmPosition":T6, "IntakeState":T2, "Claw Open":bool, "ArmOffsetTime (ms)":u16, "ClawReleaseTime (ms)":i32}
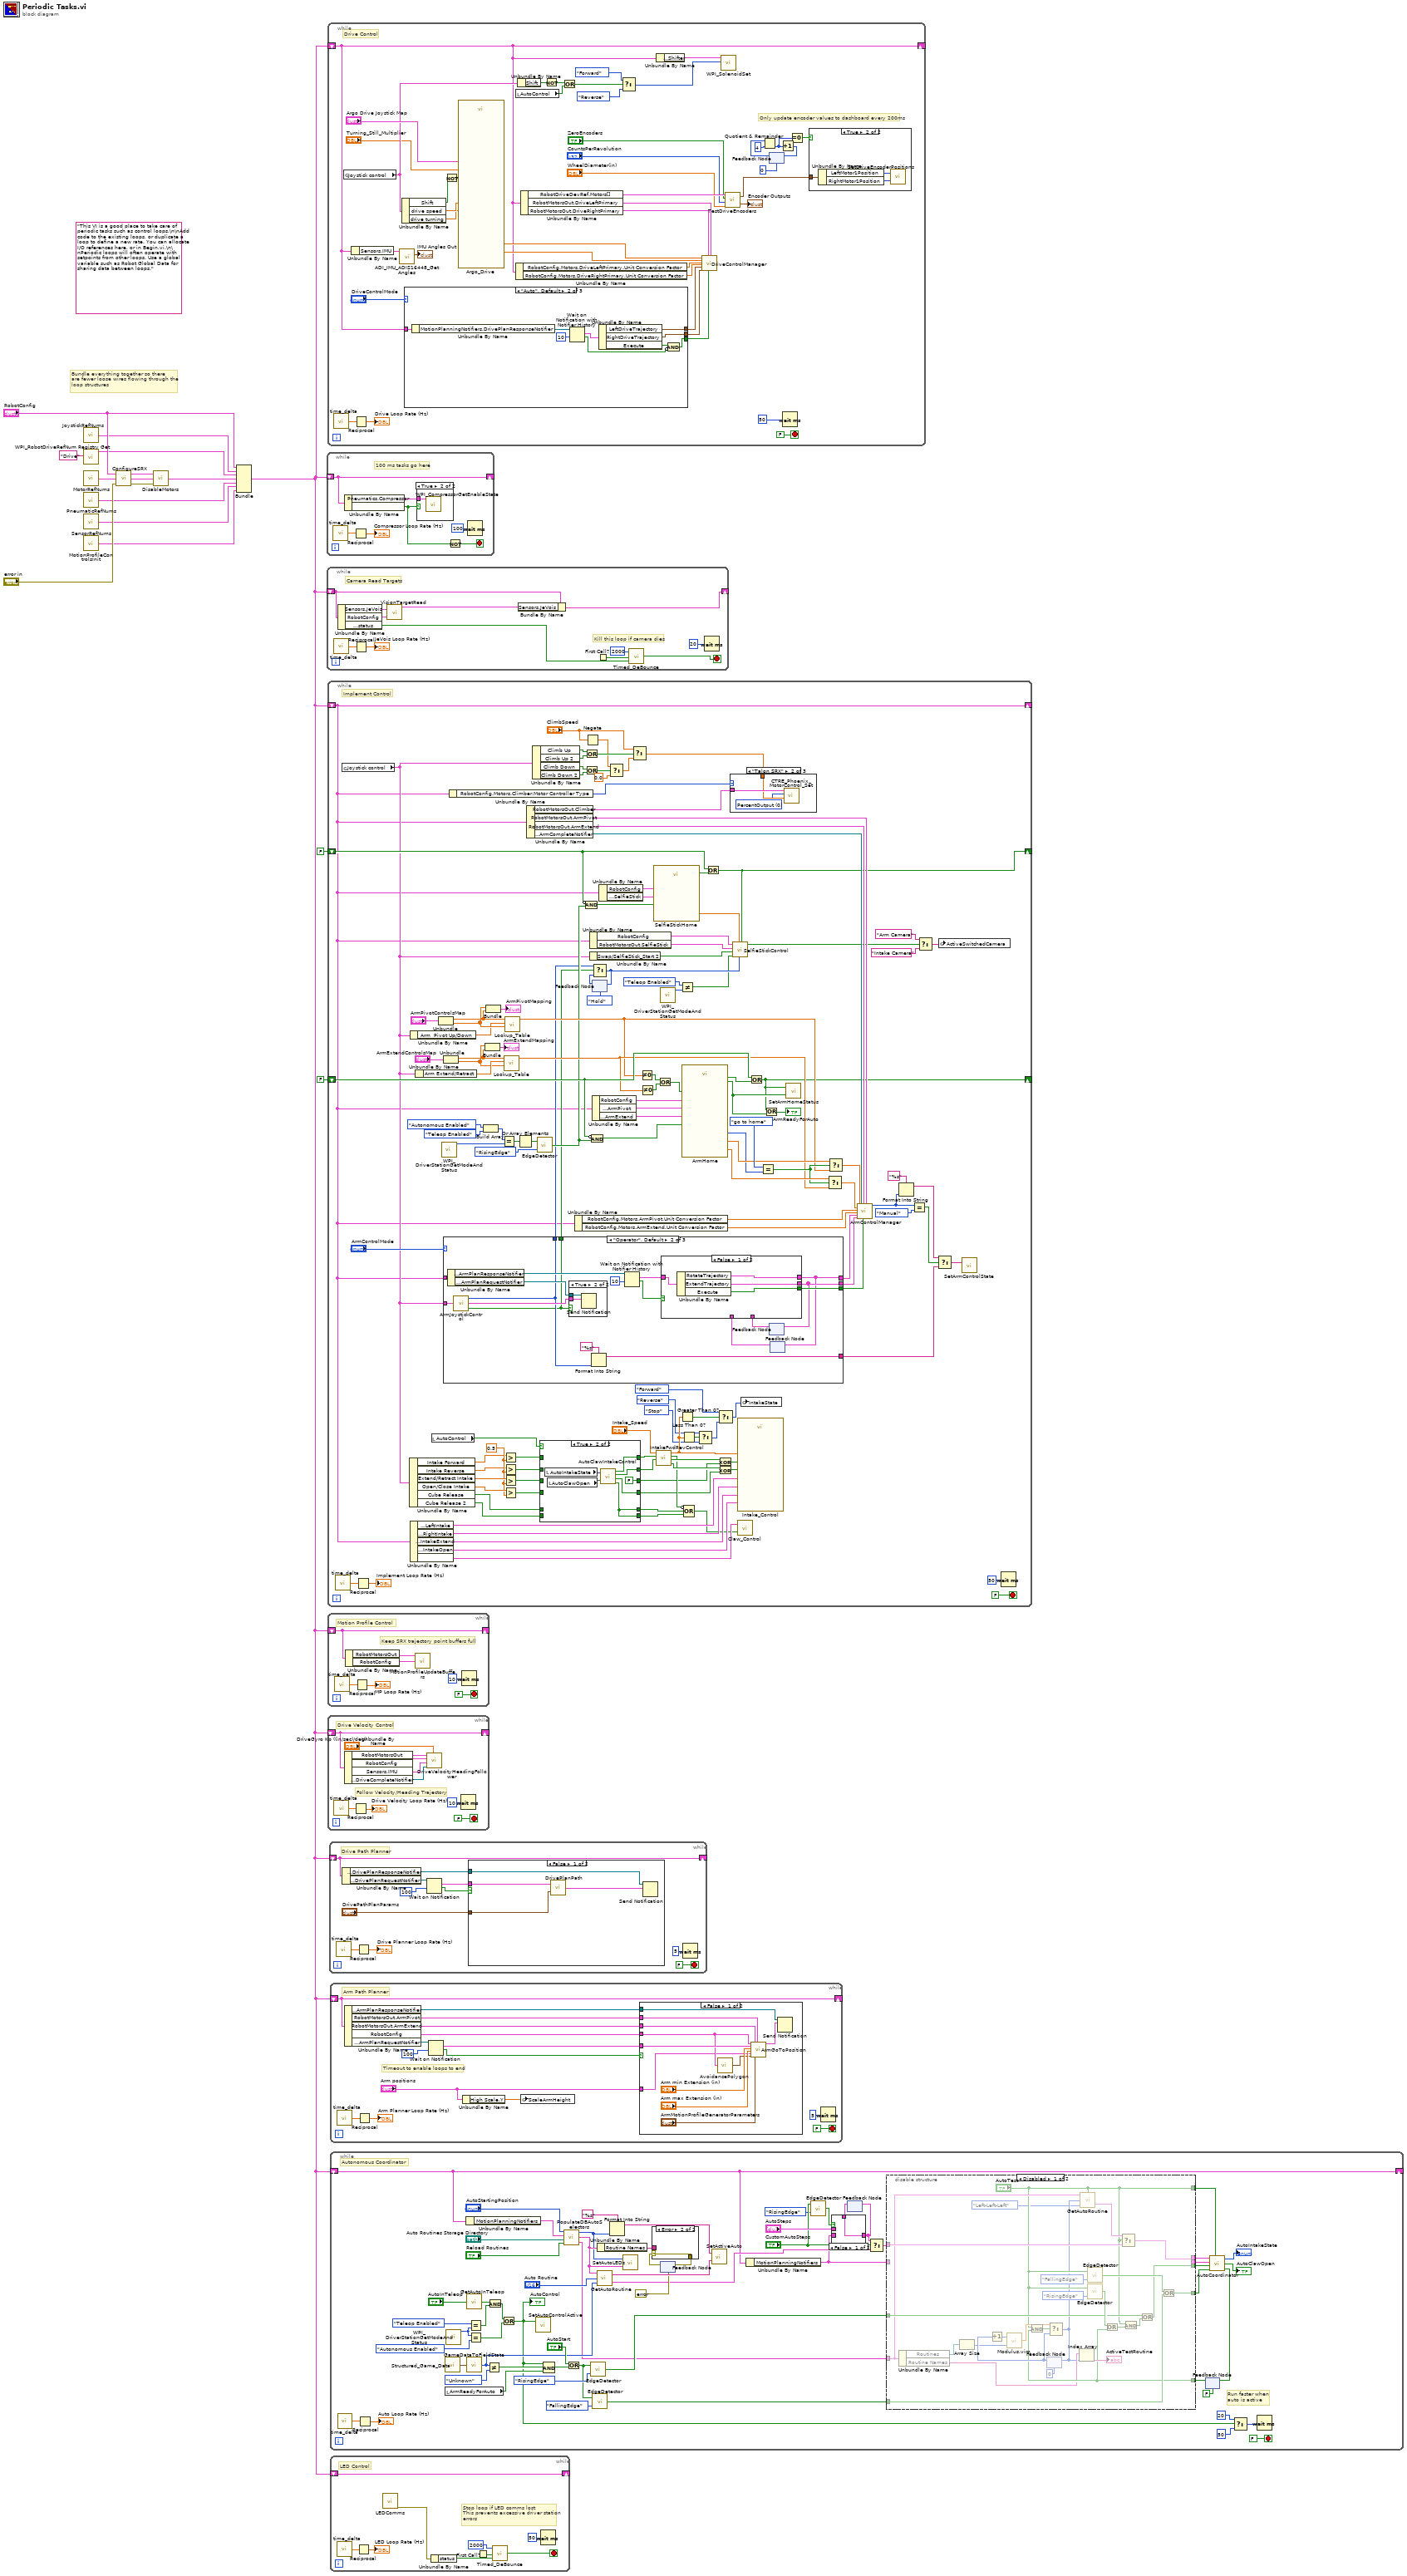
[diagram p0: block diagram]
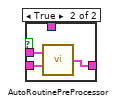
[diagram p2: hidden frame]
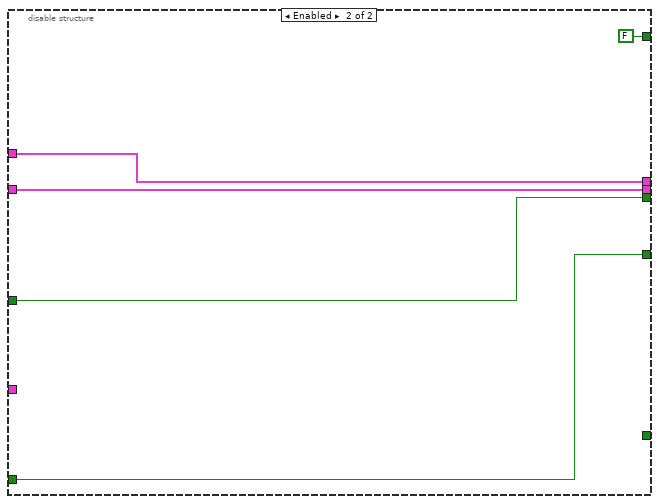
[diagram p3: hidden frame]
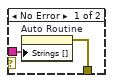
[diagram p4: hidden frame]
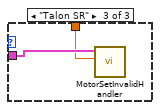
[diagram p8: hidden frame]
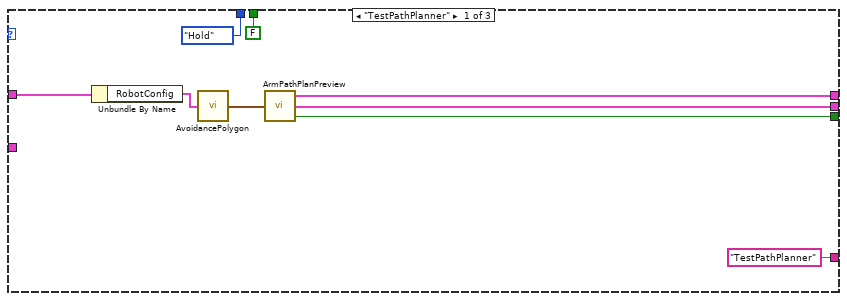
[diagram p10: hidden frame]
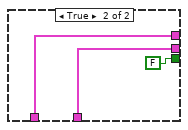
[diagram p11: hidden frame]
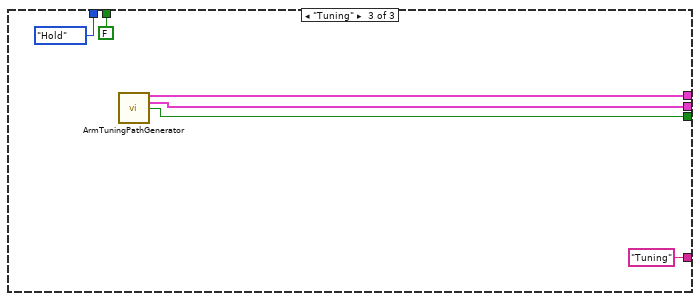
[diagram p13: hidden frame]
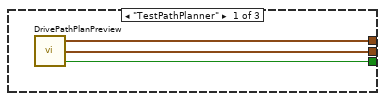
[diagram p16: hidden frame]
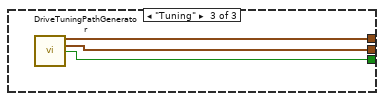
[diagram p17: hidden frame]
diagram:
  (unwired) "This VI is a good place to take care of periodic tasks such as control loops.\n\nAdd code to the existing loops, or duplicate a loop to define a new rate. You can allocate I/O references here, or in Begin.vi.\n\nPeriodic loops will often operate with setpoints from other loops. Use a global variable such as Robot Global Data for sharing data between loops."
  # "Bundle everything together so there\nare fewer loose wires flowing through the\nloop structures"
  n1 = call "JoystickRefNums.vi"() -> ("Joysticks"=w12:T35)  [unwired: 1 in]
  n2 = call <vilib>:"WPI_RobotDriveRefNum Registry Get.vi"("refnum name"="Drive") -> ("RobotDriveDevRef"=w11:T38)  [unwired: 1 in, 9 out]
  n3 = call "MotorRefNums.vi"() -> ("MotorRefNums"=w13:T42)  [unwired: 1 in]
  n4 = call "PneumaticRefNums.vi"() -> ("Pneumatics"=w9:T43)  [unwired: 1 in]
  n5 = call "SensorRefNums.vi"() -> ("Sensors"=w8:T46)  [unwired: 1 in]
  n6 = call "MotionProfileControlsInit.vi"() -> ("MotionPlanningNotifiers"=w7:T50)  [unwired: 1 in]
  n7 = call "ConfigureSRX.vi"("error in"="error in", "RobotMotors"=w13, "RobotConfig"="RobotConfig") -> ("error out"=w1:errorcluster, "RobotMotorsOut"=w10:T42, "RobotConfigOut"=w2:T17)
  n8 = call "DisableMotors.vi"("error in"=w1, "RobotMotors"=w10, "RobotConfig"=w2) -> ("RobotMotorsOut"=w3:T42)  [unwired: 2 out]
  n9 = Bundle("RobotConfig"="RobotConfig", "Joysticks"=w12, "RobotDriveDevRef"=w11, "RobotMotorsOut"=w3, "Pneumatics"=w9, "Sensors"=w8, "MotionPlanningNotifiers"=w7) -> (w5:T51)  [unwired: 1 in]
  n10 = while {
    shift-right: [w22] -> _
    shift-left: w5 -> [w22]
    stop <- w18 stop-if-true
    # "100 ms tasks go here"
    n11 = call "time_delta.vi"() -> ("dt (s)"=w19:dbl)  [unwired: 1 in]
    n12 = Unbundle By Name(w22) -> ("Pneumatics.Compressor"=w21:T45, "RobotConfig.Enable Compressor"=w17:bool)
    n13 = Reciprocal(x=w19) -> (1/x=→"Compressor Loop Rate (Hz)":dbl)
    n14 = case shown="True" w17 {
      tunnel: w21 -> [_ w24]
      frame False {
      }
      frame True {
        n15 = call <vilib>:"WPI_CompressorGetEnableState.vi"("CompressorDevRef"=w24) -> ()  [unwired: 7 in, 4 out]
      }
    }
    n16 = Not(x=w17) -> (.not. x?=w18:bool)
    n17 = Wait (ms)(milliseconds to wait=u32 100) -> ()  [unwired: 1 out]
  }
  n18 = while {
    shift-right: [w33] -> _
    shift-left: w5 -> [w34]
    stop <- w28 stop-if-true
    # "Kill this loop if camera dies"
    # "Camera Read Targets"
    n19 = call "time_delta.vi"() -> ("dt (s)"=w26:dbl)  [unwired: 1 in]
    n20 = Unbundle By Name(w34) -> ("Sensors.JeVois"=w36:T49, "RobotConfig"=w35:T17, "Sensors.JeVois.DevStatus.status"=w30:bool)
    n21 = Reciprocal(x=w26) -> (1/x=→"JeVois Loop Rate (Hz)":dbl)
    n22 = call "VisionTargetRead.vi"("RobotConfig"=w35, "JeVois Camera DevRef"=w36) -> ("JeVoisOut"=w32:T49)  [unwired: 4 out]
    n23 = Bundle By Name(cluster=w34, "Sensors.JeVois"=w32) -> (w33:T51)
    n24 = First Call?() -> (First Call?: T/F=w27:bool)
    n25 = call "Timed_DeBounce.vi"("Input"=w30, "Reset"=w27, "Hold Time(ms)"=u32 2000) -> ("Output"=w28:bool)
    n26 = Wait (ms)(milliseconds to wait=u32 20 ("f")) -> ()  [unwired: 1 out]
  }
  n27 = while {
    shift-right: [w44] -> _
    shift-left: w5 -> [w44]
    stop <- FALSE stop-if-true
    # "Drive Velocity Control"
    # "Follow Velocity/Heading Trajectory"
    n28 = call "time_delta.vi"() -> ("dt (s)"=w42:dbl)  [unwired: 1 in]
    n29 = Unbundle By Name(w44) -> ("RobotMotorsOut"=w41:T42, "RobotConfig"=w40:T17, "Sensors.IMU"=w39:T47, "MotionPlanningNotifiers.DriveCompleteNotifier"=w37:refnum<notifier>)
    n30 = Reciprocal(x=w42) -> (1/x=→"Drive Velocity Loop Rate (Hz)":dbl)
    n31 = call "DriveVelocityHeadingFollower.vi"("RobotMotors"=w41, "RobotConfig"=w40, "IMU DevRef"=w39, "DriveCompleteNotifier"=w37, "DriveGyro Kp ((in/sec)/deg)"="DriveGyro Kp ((in/sec)/deg)") -> ()  [unwired: 1 in]
    n32 = Wait (ms)(milliseconds to wait=u32 10) -> ()  [unwired: 1 out]
  }
  n33 = while {
    shift-right: [w62] -> _
    shift-left: w5 -> [w62]
    stop <- FALSE stop-if-true
    # "Only update encoder values to dashboard every 200ms"
    # "Drive Control"
    n34 = call "time_delta.vi"() -> ("dt (s)"=w64:dbl)  [unwired: 1 in]
    n35 = global read "Joystick_Control.vi" "Joystick control"() -> (w66:T53)
    n36 = Unbundle By Name(w62) -> ("Sensors.IMU"=w61:T47)
    n37 = Reciprocal(x=w64) -> (1/x=→"Drive Loop Rate (Hz)":dbl)
    n38 = call "ADI_IMU_ADIS16448_Get Angles.vi"("ADI IMU DevRef"=w61) -> ("IMU Angles Out"=→"IMU Angles Out":T9)  [unwired: 7 in, 3 out]
    n39 = Unbundle By Name(w66) -> ("Shift"=w81:bool, "drive speed"=w88:dbl, "drive turning"=w87:dbl)
    n40 = case shown="\"Auto\", Default" "DriveControlMode" {
      tunnel: [w94 w101 w108] -> w74
      tunnel: [w95 w100 w107] -> w73
      tunnel: [w96 w99 w106] -> w72
      tunnel: w62 -> [_ w105 _]
      frame "TestPathPlanner" {
        n41 = call "DrivePathPlanPreview.vi"() -> ("LeftTrajectory"=w94:T54[], "RightTrajectory"=w95:T54[], "Go"=w96:bool)  [unwired: 1 in]
      }
      frame "Auto", Default {
        n42 = Unbundle By Name(w105) -> ("MotionPlanningNotifiers.DrivePlanResponseNotifier"=w104:refnum<notifier>)
        n43 = Wait on Notification with Notifier History(0:w104, 2:10 ("timeout in ms (-1)")) -> (9:w102:T55, 10:w97:bool)  [unwired: 2 in, 2 out]
        n44 = Unbundle By Name(w102) -> ("LeftDriveTrajectory"=w101:T54[], "RightDriveTrajectory"=w100:T54[], "Execute"=w98:bool)
        n45 = Compound Arithmetic op=AND(w98, invert w97) -> (w99:bool)
      }
      frame "Tuning" {
        n46 = call "DriveTuningPathGenerator.vi"() -> ("Left Drive Motion Profile"=w108:T54[], "Right Drive Motion Profile"=w107:T54[], "Go"=w106:bool)  [unwired: 13 in]
      }
    }
    n47 = Not(x=w81) -> (.not. x?=w56:bool)
    n48 = call "Argo_Drive.vi"("Speed_Main"=w88, "Turning_Still_Multiplier"="Turning_Still_Multiplier", "Argo Drive Joystick Map"="Argo Drive Joystick Map", "Turning_Main"=w87, "High_Gear"=w56) -> ("Left_Motor"=w78:dbl, "Right_Motor"=w77:dbl)  [unwired: 13 in]
    n49 = local read "AutoControl"() -> (w57:bool)
    n50 = Unbundle By Name(w62) -> ("RobotConfig.Motors.DriveLeftPrimary.Unit Conversion Factor"=w76:dbl, "RobotConfig.Motors.DriveRightPrimary.Unit Conversion Factor"=w75:dbl)
    n51 = Unbundle By Name(w66) -> ("Shift"=w69:bool)
    n52 = Unbundle By Name(w62) -> ("RobotDriveDevRef.Motors[]"=w86:T39[], "RobotMotorsOut.DriveLeftPrimary"=w80:T39, "RobotMotorsOut.DriveRightPrimary"=w79:T39)
    n53 = Not(x=w69) -> (.not. x?=w55:bool)
    n54 = Or(x=w55, y=w57) -> (x .or. y?=w58:bool)
    n55 = Select(t=WPI_SolenoidValue."Forward" ("Value"), s=w58, f=WPI_SolenoidValue."Reverse" ("Value")) -> (s? t:f=w68:T52)
    n56 = Unbundle By Name(w62) -> ("Pneumatics.Shifter"=w67:T44)
    n57 = call "DriveControlManager.vi"("Left Drive Manual Control"=w78, "Right Drive Manual Control"=w77, "left drive unit conversion (ticks/in)"=w76, "right drive unit coversion (ticks/in)"=w75, "LeftTrajectory"=w74, "RightTrajectory"=w73, "Right Drive Motor DevRef"=w79, "New Motion Profile"=w72, "Left Drive Motor DevRef"=w80) -> ()  [unwired: 10 in, 1 out]
    n58 = call-poly <vilib>:"WPI_SolenoidSet.vi"("Value"=w68, "SolenoidDevRef"=w67) -> ()  [unwired: 8 in, 2 out]
    n59 = call "TestDriveEncoders.vi"("WheelDiameter(in)"="WheelDiameter(in)", "CountsPerRevolution"="CountsPerRevolution", "ZeroSensors"="ZeroEncoders", "RobotDriveMotors"=w86) -> ("Drive Encoder Outputs"=→"Encoder Outputs":T56, "Drive Encoder Outputs Raw"=w53:T57)
    n60 = feedback #1(u8 0) -> (w50:u8)
    n61 = Quotient & Remainder(x=w50, y=u8 4) -> (floor(x/y)=w48:u8)  [unwired: 1 out]
    n62 = Increment(x=w48) -> (x+1=w47:u8)
    n63 = feedback-in #1(w47) -> ()
    n64 = Wait (ms)(milliseconds to wait=u32 50) -> ()  [unwired: 1 out]
    n65 = Equal To 0?(x=w48) -> (x = 0?=w51:bool)
    n66 = case shown="True" w51 {
      tunnel: w53 -> [_ w93]
      frame False {
      }
      frame True {
        n67 = Unbundle By Name(w93) -> ("LeftMotor1Position"=w92:i32, "RightMotor1Position"=w91:i32)
        n68 = call "SetDriveEncoderPositions.vi"("DriveEncoderRight"=w91, "DriveEncoderLeft"=w92) -> ()  [unwired: 1 in]
      }
    }
  }
  n69 = while {
    shift-right: [w110] -> _
    shift-left: w5 -> [w110]
    shift-right: [w136] -> _
    shift-left: FALSE -> [w204]
    shift-right: [w119] -> _
    shift-left: FALSE -> [w130]
    stop <- FALSE stop-if-true
    w200 = 0.5 ("y")
    # "Implement Control"
    n70 = call "time_delta.vi"() -> ("dt (s)"=w172:dbl)  [unwired: 1 in]
    n71 = global read "Joystick_Control.vi" "Joystick control"() -> (w117:T53)
    n72 = Reciprocal(x=w172) -> (1/x=→"Implement Loop Rate (Hz)":dbl)
    n73 = Unbundle By Name(w117) -> ("Intake Forward"=w199:dbl, "Intake Reverse"=w198:dbl, "Extend/Retract Intake"=w202:dbl, "Open/Close Intake"=w201:dbl, "Cube Release"=w162:bool, "Cube Release 2"=w161:bool)
    n74 = Unbundle By Name(w117) -> ("Arm  Pivot Up/Down"=w168:dbl)
    n75 = Unbundle By Name(w110) -> ("RobotMotorsOut.LeftIntake"=w192:T39, "RobotMotorsOut.RightIntake"=w193:T39, "Pneumatics.IntakeExtend"=w194:T44, "Pneumatics.IntakeOpen"=w195:T44, "Pneumatics.ArmClaw"=w196:T44)
    n76 = Unbundle By Name(w117) -> ("Arm Extend/Retract"=w220:dbl)
    n77 = local read "AutoControl"() -> (w145:bool)
    n78 = Unbundle("ArmPivotControlsMap") -> ("Look Up Table OUT"=w215:dbl[], "Look Up Table IN"=w217:dbl[])
    n79 = call <vilib>:"WPI_DriverStationGetModeAndStatus.vi"() -> ("Robot Mode"=w208:T58)  [unwired: 10 in, 1 out]
    n80 = Unbundle("ArmExtendControlsMap") -> ("Look Up Table OUT"=w213:dbl[], "Look Up Table IN"=w214:dbl[])
    n81 = case shown="\"Operator\", Default" "ArmControlMode" {
      tunnel: [w267 w276 w301] -> w240
      tunnel: [w268 w277 w300] -> w239
      tunnel: [w269 w278 w299] -> w238
      tunnel: w110 -> [w265 w285 _]
      tunnel: w117 -> [_ w286 _]
      tunnel: ["TestPathPlanner" w272 "Tuning"] -> w140
      tunnel: [ArmTargetPosition."Hold" ("TargetPosition") w271 ArmTargetPosition."Hold" ("TargetPosition")] -> w124
      tunnel: [FALSE ("NewPath") w270 FALSE ("NewPath")] -> w123
      frame "TestPathPlanner" {
        n82 = Unbundle By Name(w265) -> ("RobotConfig"=w264:T17)
        n83 = call "AvoidancePolygon.vi"("RobotConfig"=w264) -> ("Polygon"=w266:T62)
        n84 = call "ArmPathPlanPreview.vi"("AvoidancePolygon"=w266) -> ("Rotation Path"=w267:T63[], "Extension Path"=w268:T63[], "Go"=w269:bool)
      }
      frame "Operator", Default {
        n85 = Unbundle By Name(w285) -> ("MotionPlanningNotifiers.ArmPlanResponseNotifier"=w282:refnum<notifier>, "MotionPlanningNotifiers.ArmPlanRequestNotifier"=w284:refnum<notifier>)
        n86 = call "ArmJoystickControl.vi"("Joystick control"=w286) -> ("TargetPosition"=w271:T6, "ArmPlanRequest"=w283:T64, "NewPath"=w270:bool)
        n87 = case shown="True" w270 {
          tunnel: w284 -> [_ w295]
          tunnel: w283 -> [_ w294]
          frame False {
          }
          frame True {
            n88 = Send Notification(notification=w294, notifier=w295) -> ()  [unwired: 1 in, 2 out]
          }
        }
        n89 = Format Into String(format string="%s", w271) -> (resulting string=w272:string)  [unwired: 2 in, 1 out]
        n90 = Wait on Notification with Notifier History(0:w282, 2:10 ("timeout in ms (-1)")) -> (9:w279:T65, 10:w280:bool)  [unwired: 2 in, 2 out]
        n91 = feedback #2() -> (w275:T63[])  [unwired: 1 in]
        n92 = feedback #3() -> (w274:T63[])  [unwired: 1 in]
        n93 = case shown="False" w280 {
          tunnel: w279 -> [w290 _]
          tunnel: [w289 w291] -> w276
          tunnel: [w288 w292] -> w277
          tunnel: [w287 FALSE ("Execute")] -> w278
          tunnel: w275 -> [_ w292]
          tunnel: w274 -> [_ w291]
          frame False {
            n94 = Unbundle By Name(w290) -> ("RotateTrajectory"=w289:T63[], "ExtendTrajectory"=w288:T63[], "Execute"=w287:bool)
          }
          frame True {
          }
        }
        n95 = feedback-in #2(w277) -> ()
        n96 = feedback-in #3(w276) -> ()
      }
      frame "Tuning" {
        n97 = call "ArmTuningPathGenerator.vi"() -> ("Rotation Motion Profile"=w301:T63[], "Extension Motion Profile"=w300:T63[], "Go"=w299:bool)  [unwired: 13 in]
      }
    }
    n98 = Unbundle By Name(w110) -> ("RobotConfig.Motors.Climber.Motor Controller Type"=w109:T22)
    n99 = Build Array(WPI_DriverStationRobotMode2."Autonomous Enabled" ("Robot Mode"), WPI_DriverStationRobotMode2."Teleop Enabled" ("Robot Mode")) -> (w209:T58[])
    n100 = Bundle("Look Up Table IN"=w214, "Look Up Table OUT"=w213) -> (→"ArmExtendMapping":T66)  [unwired: 1 in]
    n101 = Bundle("Look Up Table IN"=w217, "Look Up Table OUT"=w215) -> (→"ArmPivotMapping":T66)  [unwired: 1 in]
    n102 = Equal?(x=w209, y=w208) -> (x = y?=w207:bool[])
    n103 = Greater?(x=w199, y=w200) -> (0:w166:bool)
    n104 = Greater?(x=w198, y=w200) -> (0:w165:bool)
    n105 = Greater?(x=w202, y=w200) -> (0:w164:bool)
    n106 = Greater?(x=w201, y=w200) -> (0:w163:bool)
    n107 = call "Lookup_Table.vi"("Y_Array"=w213, "x_in"=w220, "X_Array"=w214) -> ("y_out"=w170:dbl)  [unwired: 6 in]
    n108 = call "Lookup_Table.vi"("Y_Array"=w215, "x_in"=w168, "X_Array"=w217) -> ("y_out"=w169:dbl)  [unwired: 6 in]
    n109 = Or Array Elements(Boolean array=w207) -> (logical OR=w206:bool)
    n110 = Unbundle By Name(w110) -> ("RobotMotorsOut.Climber"=w185:T39, "RobotMotorsOut.ArmPivot"=w236:T39, "RobotMotorsOut.ArmExtend"=w235:T39, "MotionPlanningNotifiers.ArmCompleteNotifier"=w167:refnum<notifier>)
    n111 = Unbundle By Name(w117) -> ("Climb Up"=w181:bool, "Climb Up 2"=w182:bool, "Climb Down"=w184:bool, "Climb Down 2"=w183:bool)
    n112 = call "EdgeDetector.vi"("DetectorType"=EdgeDetector_Type."RisingEdge", "Input"=w206) -> ("Edge"=w131:bool)
    n113 = case shown="True" w145 {
      tunnel: w166 -> [w251 _]
      tunnel: w165 -> [w250 _]
      tunnel: w164 -> [w249 _]
      tunnel: w163 -> [w248 _]
      tunnel: w162 -> [w253 _]
      tunnel: w161 -> [w252 _]
      tunnel: [w253 w255] -> w160
      tunnel: [w252 w255] -> w159
      tunnel: [w251 w258] -> w158
      tunnel: [w250 w257] -> w157
      tunnel: [w249 FALSE] -> w156
      tunnel: [w248 w256] -> w155
      frame False {
      }
      frame True {
        n114 = local read "AutoIntakeState"() -> (w259:T2)
        n115 = local read "AutoClawOpen"() -> (w260:bool)
        n116 = call "AutoClawIntakeControl.vi"("IntakeState"=w259, "ClawOpen"=w260) -> ("Intake Forward"=w258:bool, "Intake Reverse"=w257:bool, "Open/Close Intake"=w256:bool, "Cube Release"=w255:bool)
      }
    }
    n117 = Unbundle By Name(w110) -> ("RobotConfig.Motors.ArmPivot.Unit Conversion Factor"=w234:dbl, "RobotConfig.Motors.ArmExtend.Unit Conversion Factor"=w233:dbl)
    n118 = Or(x=w181, y=w182) -> (x .or. y?=w178:bool)
    n119 = Or(x=w184, y=w183) -> (x .or. y?=w180:bool)
    n120 = Negate(x="ClimbSpeed") -> (-x=w175:dbl)
    n121 = Compound Arithmetic op=AND(invert w130, w131) -> (w132:bool)
    n122 = Unbundle By Name(w110) -> ("RobotConfig"=w116:T17, "RobotMotorsOut.SelfieStick"=w115:T39)
    n123 = Unbundle By Name(w117) -> ("Swap/SelfieStick_Start 2"=w112:bool)
    n124 = Compound Arithmetic op=AND(invert w204, w131) -> (w203:bool)
    n125 = feedback #4(ArmTargetPosition."Hold" ("TargetPosition")) -> (w125:T6)
    n126 = Unbundle By Name(w110) -> ("RobotConfig"=w226:T17, "RobotMotorsOut.ArmPivot"=w225:T39, "RobotMotorsOut.ArmExtend"=w224:T39)
    n127 = Select(t=w124, s=w123, f=w125) -> (s? t:f=w121:T6)
    n128 = feedback-in #4(w121) -> ()
    n129 = Unbundle By Name(w110) -> ("RobotConfig"=w134:T17, "RobotMotorsOut.SelfieStick"=w129:T39)
    n130 = Select(t=w175, s=w180, f=0.0) -> (s? t:f=w179:dbl)
    n131 = Select(t="ClimbSpeed", s=w178, f=w179) -> (s? t:f=w174:dbl)
    n132 = Not Equal To 0?(x=w169) -> (x != 0?=w222:bool)
    n133 = Not Equal To 0?(x=w170) -> (x != 0?=w223:bool)
    n134 = call "SelfieStickHome.vi"("Selfie Stick Motor DevRef"=w129, "RobotConfig"=w134, "Start"=w132) -> ("Selfie Stick Motor Speed"=w120:dbl, "Complete"=w133:bool)  [unwired: 9 in, 2 out]
    n135 = call "IntakeFwdRevControl.vi"("Intake Reverse"=w157, "Intake Forward"=w158, "IntakeMaxSpeed"="Intake_Speed") -> ("IntakeOpen"=w188:bool, "IntakeExtend"=w189:bool, "ClawClose"=w186:bool, "Intake Speed"=w154:dbl)  [unwired: 1 in]
    n136 = Or(x=w222, y=w223) -> (x .or. y?=w221:bool)
    n137 = call <vilib>:"WPI_DriverStationGetModeAndStatus.vi"() -> ("Robot Mode"=w114:T58)  [unwired: 10 in, 1 out]
    n138 = Not Equal?(x=WPI_DriverStationRobotMode2."Teleop Enabled", y=w114) -> (x != y?=w111:bool)
    n139 = Greater Than 0?(x=w154) -> (x > 0?=w153:bool)
    n140 = Less Than 0?(x=w154) -> (x < 0?=w152:bool)
    n141 = call "ArmHome.vi"("arm rotate motor devref"=w225, "RobotConfig"=w226, "arm extend motor devref"=w224, "start"=w203, "stop"=w221) -> ("arm rotate speed"=w231:dbl, "arm extend speed"=w230:dbl, "complete"=w146:bool, "failed"=w137:bool, "arm homing state"=w173:T61)  [unwired: 6 in]
    n142 = Compound Arithmetic op=OR(invert w186, w160, w159) -> (w187:bool)
    n143 = Select(t=IntakeState."Reverse" ("IntakeState"), s=w152, f=IntakeState."Stop" ("IntakeState")) -> (s? t:f=w151:T2)
    n144 = Or(x=w130, y=w133) -> (x .or. y?=w119:bool)
    n145 = Select(t=IntakeState."Forward" ("IntakeState"), s=w153, f=w151) -> (s? t:f=w150:T2)
    n146 = Exclusive Or(1:w156, 2:w189) -> (0:w190:bool)
    n147 = Exclusive Or(1:w155, 2:w188) -> (0:w191:bool)
    n148 = case shown="\"Talon SRX\"" w109 {
      tunnel: w185 -> [_ w245 w247]
      tunnel: w174 -> [_ w244 w246]
      frame "Disabled", Default {
      }
      frame "Talon SRX" {
        w243 = T67 0 items=["PercentOutput"=0, "Position"=1, "Velocity"=2, "Current"=3, "Follower"=5, "MotionProfile"=6, "MotionMagic"=7, "MotionMagicArc"=8, "MotionProfileArc"=10, "Disabled"=15] ("Control Mode")
        n149 = call <vilib>:"CTRE_Phoenix_MotorControl_Set.vi"("Output"=w244, "Control Mode"=w243, "PhoenixMotorControlDevRef"=w245) -> ()  [unwired: 7 in, 2 out]
      }
      frame "Talon SR" {
        n150 = call "MotorSetInvalidHandler.vi"("Output"=w246, "MotorControlDevRef"=w247) -> ()  [unwired: 7 in, 3 out]
      }
    }
    n151 = call "SelfieStickControl.vi"("Home Complete"=w119, "Arm Position"=w121, "Manual Control"=w120, "Inhibit Extend"=w111, "Manual Toggle"=w112, "Selfie Stick Motor DevRef"=w115, "RobotConfig"=w116) -> ("Use Arm Camera"=w118:bool)  [unwired: 3 in, 1 out]
    n152 = call "Intake_Control.vi"("LeftIntakeDevRef"=w192, "RightIntakeDevRef"=w193, "IntakeExtendDevRef"=w194, "IntakeOpenDevRef"=w195, "IntakeExtend"=w190, "IntakeOpen"=w191, "IntakeSpeed"=w154) -> ()  [unwired: 13 in]
    n153 = call "Claw_Control.vi"("Claw Open"=w187, "Claw_Solenoid"=w196) -> ()  [unwired: 1 in]
    n154 = global write "LEDData.vi" "IntakeState"(w150) -> ()
    n155 = Or(x=w204, y=w146) -> (x .or. y?=w136:bool)
    n156 = Equal?(x=ArmHomingState."go to home", y=w173) -> (x = y?=w229:bool)
    n157 = Or(x=w136, y=w137) -> (x .or. y?=→"ArmReadyForAuto":bool)
    n158 = call "SetArmHomeStatus.vi"("ArmHomeFailure"=w137, "ArmHomeSuccess"=w136) -> ()  [unwired: 1 in]
    n159 = Select(t=w230, s=w229, f=w170) -> (s? t:f=w228:dbl)
    n160 = Select(t=w231, s=w229, f=w169) -> (s? t:f=w227:dbl)
    n161 = call "ArmControlManager.vi"("Arm Rotate Manual Control"=w227, "Arm Extend Manual Control"=w228, "rotate sensor unit conversion (ticks/rad)"=w234, "extend sensor unit coversion (ticks/in)"=w233, "Arm Rotate Motion Profile"=w240, "Arm Extend Motion Profile"=w239, "ArmCompleteNotifier"=w167, "Arm Extend Motor DevRef"=w235, "New Motion Profile"=w238, "Arm Rotate Motor DevRef"=w236) -> ("Arm Control State"=w142:T59)  [unwired: 9 in]
    n162 = Format Into String(format string="%s", w142) -> (resulting string=w139:string)  [unwired: 2 in, 1 out]
    n163 = Equal?(x=w142, y=MotionProfileControlState."Manual") -> (x = y?=w141:bool)
    n164 = Select(t="Arm Camera", s=w118, f="Intake Camera") -> (s? t:f=w128:string)
    n165 = Select(t=w139, s=w141, f=w140) -> (s? t:f=w138:string)
    n166 = global write "SwitchedCameraData.vi" "ActiveSwitchedCamera"(w128) -> ()
    n167 = call "SetArmControlState.vi"("ArmControlState"=w138) -> ()  [unwired: 2 in]
    n168 = Wait (ms)(milliseconds to wait=u32 50) -> ()  [unwired: 1 out]
  }
  n169 = while {
    shift-right: [w306] -> _
    shift-left: w5 -> [w306]
    stop <- FALSE stop-if-true
    # "Motion Profile Control"
    # "Keep SRX trajectory point buffers full"
    n170 = call "time_delta.vi"() -> ("dt (s)"=w302:dbl)  [unwired: 1 in]
    n171 = Unbundle By Name(w306) -> ("RobotMotorsOut"=w305:T42, "RobotConfig"=w304:T17)
    n172 = Reciprocal(x=w302) -> (1/x=→"MP Loop Rate (Hz)":dbl)
    n173 = call "MotionProfileUpdateBuffers.vi"("RobotConfig"=w304, "RobotMotors"=w305) -> ()  [unwired: 1 in, 3 out]
    n174 = Wait (ms)(milliseconds to wait=u32 10) -> ()  [unwired: 1 out]
  }
  n175 = while {
    shift-right: [w317] -> _
    shift-left: w5 -> [w317]
    stop <- FALSE stop-if-true
    # "Drive Path Planner"
    n176 = call "time_delta.vi"() -> ("dt (s)"=w311:dbl)  [unwired: 1 in]
    n177 = Unbundle By Name(w317) -> ("MotionPlanningNotifiers.DrivePlanResponseNotifier"=w312:refnum<notifier>, "MotionPlanningNotifiers.DrivePlanRequestNotifier"=w316:refnum<notifier>)
    n178 = Reciprocal(x=w311) -> (1/x=→"Drive Planner Loop Rate (Hz)":dbl)
    n179 = Wait on Notification(notifier=w316, timeout in ms (-1)=100) -> (notification=w313:T68, timed out?=w314:bool)  [unwired: 2 in, 2 out]
    n180 = case shown="False" w314 {
      tunnel: w313 -> [w322 _]
      tunnel: w312 -> [w323 _]
      tunnel: "DrivePathPlanParams" -> [w320 _]
      frame False {
        n181 = call "DrivePlanPath.vi"("DrivePathPlanParams"=w320, "DrivePlanRequest"=w322) -> ("DrivePlanResponse"=w321:T55)
        n182 = Send Notification(notification=w321, notifier=w323) -> ()  [unwired: 1 in, 2 out]
      }
      frame True {
        # "Timeout"
      }
    }
    n183 = Wait (ms)(milliseconds to wait=u32 5) -> ()  [unwired: 1 out]
  }
  n184 = while {
    shift-right: [w336] -> _
    shift-left: w5 -> [w336]
    stop <- FALSE stop-if-true
    # "Timeout to enable loops to end"
    # "Arm Path Planner"
    n185 = call "time_delta.vi"() -> ("dt (s)"=w326:dbl)  [unwired: 1 in]
    n186 = Unbundle By Name(w336) -> ("MotionPlanningNotifiers.ArmPlanResponseNotifier"=w332:refnum<notifier>, "RobotMotorsOut.ArmPivot"=w330:T39, "RobotMotorsOut.ArmExtend"=w329:T39, "RobotConfig"=w328:T17, "MotionPlanningNotifiers.ArmPlanRequestNotifier"=w331:refnum<notifier>)
    n187 = Reciprocal(x=w326) -> (1/x=→"Arm Planner Loop Rate (Hz)":dbl)
    n188 = Wait on Notification(notifier=w331, timeout in ms (-1)=100) -> (notification=w333:T64, timed out?=w334:bool)  [unwired: 2 in, 2 out]
    n189 = Unbundle By Name("Arm positions") -> ("High Scale.Y"=w324:dbl)
    n190 = global write "LEDData.vi" "ScaleArmHeight"(w324) -> ()
    n191 = case shown="False" w334 {
      tunnel: w333 -> [w344 _]
      tunnel: w332 -> [w349 _]
      tunnel: w330 -> [w342 _]
      tunnel: w329 -> [w341 _]
      tunnel: w328 -> [w340 _]
      tunnel: "Arm positions" -> [w339 _]
      frame False {
        n192 = call "AvoidancePolygon.vi"("RobotConfig"=w340) -> ("Polygon"=w345:T62)
        n193 = call "ArmGoToPosition.vi"("RobotConfig"=w340, "ArmPlanRequest"=w344, "Arm min Extension (in)"="Arm min Extension (in)", "Arm max Extension (in)"="Arm max Extension (in)", "Arm positions"=w339, "Avoidance Polygon"=w345, "Arm extend motor"=w341, "MotionProfileGeneratorParameters"="ArmMotionProfileGeneratorParameters", "Arm rotate motor"=w342) -> ("ArmPlanResponse"=w343:T65)  [unwired: 10 in]
        n194 = Send Notification(notification=w343, notifier=w349) -> ()  [unwired: 1 in, 2 out]
      }
      frame True {
        # "Timeout"
      }
    }
    n195 = Wait (ms)(milliseconds to wait=u32 5) -> ()  [unwired: 1 out]
  }
  n196 = while {
    shift-right: [w352] -> _
    shift-left: w5 -> [w352]
    stop <- FALSE stop-if-true
    # "Run faster when\nauto is active"
    # "Autonomous Coordinator"
    n197 = call "time_delta.vi"() -> ("dt (s)"=w410:dbl)  [unwired: 1 in]
    n198 = Reciprocal(x=w410) -> (1/x=→"Auto Loop Rate (Hz)":dbl)
    n199 = call "Structured_Game_Data.vi"() -> ("Game Data"=w405:T70)  [unwired: 1 in]
    n200 = local read "ArmReadyForAuto"() -> (w403:bool)
    n201 = call <vilib>:"WPI_DriverStationGetModeAndStatus.vi"() -> ("Robot Mode"=w392:T58)  [unwired: 10 in, 1 out]
    n202 = Unbundle By Name(w352) -> ("MotionPlanningNotifiers"=w351:T50)
    n203 = call "GetAutoInTeleop.vi"("AutoInTeleopOverride"="AutoInTeleop") -> ("AutoInTeleop"=w389:bool)
    n204 = call "GameDataToFieldState.vi"("Game Data"=w405) -> ("FieldState"=w394:T69)
    n205 = Equal?(x=WPI_DriverStationRobotMode2."Teleop Enabled", y=w392) -> (x = y?=w388:bool)
    n206 = Equal?(x=w392, y=WPI_DriverStationRobotMode2."Autonomous Enabled" ("x")) -> (x = y?=w386:bool)
    n207 = Not Equal?(x=w394, y=AutoFieldState."Unknown") -> (x != y?=w402:bool)
    n208 = And(x=w389, y=w388) -> (x .and. y?=w387:bool)
    n209 = Or(x=w387, y=w386) -> (x .or. y?=w375:bool)
    "AutoControl" <- w375
    n210 = call "SetAutoControlActive.vi"("AutoControlActive"=w375) -> ()  [unwired: 2 in]
    n211 = Compound Arithmetic op=AND(w375, w402, w403) -> (w401:bool)
    n212 = call "PopulateDBAutoSelectors.vi"("Reload Routines"="Reload Routines", "Auto Routines Storage Directory"="Auto Routines Storage Directory", "MotionPlanningNotifiers"=w351, "DefaultStartingPosition"="AutoStartingPosition") -> ("AllRoutines"=w350:T72, "AvailableRoutines"=w373:T72, "StartingPosition"=w372:T1)
    n213 = Or(x="AutoStart", y=w401) -> (x .or. y?=w385:bool)
    n214 = call "EdgeDetector.vi"("DetectorType"=EdgeDetector_Type."RisingEdge", "Input"=w385) -> ("Edge"=w370:bool)
    n215 = call "EdgeDetector.vi"("DetectorType"=EdgeDetector_Type."FallingEdge", "Input"=w385) -> ("Edge"=w371:bool)
    n216 = Unbundle By Name(w373) -> ("Routine Names"=w406:string[])
    n217 = call "GetAutoRoutine.vi"("FieldState"=w394, "Default Auto Routine"="Auto Routine", "AvailableRoutines"=w373) -> ("Selected Routine"=w374:T73[], "Selected Routine Name"=w383:string)  [unwired: 1 in]
    n218 = Format Into String(format string="%s", w372) -> (resulting string=w381:string)  [unwired: 2 in, 1 out]
    n219 = call "SetAutoLEDs.vi"("AvailableRoutines"=w373, "AutoStartingPosition"=w372) -> ()  [unwired: 1 in]
    n220 = feedback #5(errorcluster {"status"=FALSE, "code"=0, "source"=""} ("error IO")) -> (w379:errorcluster)
    n221 = case shown="Error" w379 {
      selector: w379 -> [_ w450]
      tunnel: w406 -> [w449 _]
      tunnel: [w448 w450] -> w380
      frame No Error {
        n222 = property on="Auto Routine" class="Ring (strict)"("Strings []"=w449) -> (error out=w448:errorcluster)  [unwired: 2 in, 1 out]
      }
      frame Error {
      }
    }
    n223 = feedback-in #5(w380) -> ()
    n224 = call "SetActiveAuto.vi"("ActiveAutoRoutine"=w383, "ActiveStartPosition"=w381) -> ()  [unwired: 1 in]
    n225 = Unbundle By Name(w352) -> ("MotionPlanningNotifiers"=w359:T50)
    n226 = call "EdgeDetector.vi"("DetectorType"=EdgeDetector_Type."RisingEdge", "Input"="CustomAutoSteps") -> ("Edge"=w357:bool)
    n227 = feedback #6() -> (w353:T73[])  [unwired: 1 in]
    n228 = case shown="False" w357 {
      tunnel: [w412 w415] -> w354
      tunnel: w359 -> [_ w414]
      tunnel: "AutoSteps" -> [_ w413]
      tunnel: w353 -> [w412 _]
      frame False {
      }
      frame True {
        n229 = call "AutoRoutinePreProcessor.vi"("MotionPlanningNotifiers"=w414, "RawSteps"=w413) -> ("PreProcessedSteps"=w415:T73[])
      }
    }
    n230 = feedback-in #6(w354) -> ()
    n231 = Select(t=w354, s="CustomAutoSteps", f=w374) -> (s? t:f=w369:T73[])
    n232 = feedback #7(FALSE ("Done")) -> (w361:bool)
    n233 = disable-structure shown="Disabled" {
      disable-tunnel: w361 -> [w424 _]
      disable-tunnel: w371 -> [w438 w443]
      disable-tunnel: [w436 w443] -> w367
      disable-tunnel: w370 -> [w434 w444]
      disable-tunnel: [w433 w444] -> w366
      disable-tunnel: w369 -> [w427 w445]
      disable-tunnel: [w426 w445] -> w364
      disable-tunnel: ["AutoTest" FALSE ("AutoTest")] -> w363
      disable-tunnel: w359 -> [_ w447]
      disable-tunnel: [_ w447] -> w365
      disable-tunnel: w350 -> [w420 _]
      frame Disabled {
        n234 = Unbundle By Name(w420) -> ("Routines"=w423:path[], "Routine Names"=w422:string[])
        n235 = Array Size(array=w423) -> (size(s)=w419:i32)
        n236 = And(x="AutoTest", y=w424) -> (x .and. y?=w442:bool)
        n237 = feedback #8(u16 0) -> (w430:u16)
        n238 = Increment(x=w430) -> (x+1=w429:u16)
        n239 = call "Modulus.vim"("y"=w419, "x"=w429) -> ("x%y"=w428:dbl)
        n240 = Select(t=w428, s=w442, f=w430) -> (s? t:f=w417:u16)
        n241 = feedback-in #8(w417) -> ()
        n242 = Index Array(array=w422, index=w417) -> (element=→"ActiveTestRoutine":string)
        n243 = call "GetAutoRoutine.vi"("Test"="AutoTest", "FieldState"=AutoFieldState."Left-Left-Left", "Default Auto Routine"=w417, "AvailableRoutines"=w420) -> ("Selected Routine"=w421:T73[])  [unwired: 1 out]
        n244 = call "EdgeDetector.vi"("DetectorType"=EdgeDetector_Type."FallingEdge", "Input"="AutoTest") -> ("Edge"=w437:bool)
        n245 = call "EdgeDetector.vi"("DetectorType"=EdgeDetector_Type."RisingEdge", "Input"="AutoTest") -> ("Edge"=w440:bool)
        n246 = Or(x=w440, y=w424) -> (x .or. y?=w435:bool)
        n247 = Select(t=w421, s="AutoTest", f=w427) -> (s? t:f=w426:T73[])
        n248 = And(x="AutoTest", y=w435) -> (x .and. y?=w432:bool)
        n249 = Or(x=w434, y=w432) -> (x .or. y?=w433:bool)
        n250 = Or(x=w437, y=w438) -> (x .or. y?=w436:bool)
      }
      frame Enabled {
      }
    }
    n251 = call "AutoCoordinator.vi"("Steps"=w364, "Test"=w363, "MotionPlanningNotifiers"=w365, "Start"=w366, "Stop"=w367) -> ("IntakeState"=→"AutoIntakeState":T2, "Claw Open"=→"AutoClawOpen":bool, "Done"=w362:bool)  [unwired: 1 in]
    n252 = feedback-in #7(w362) -> ()
    n253 = Select(t=u32 20, s=w375, f=u32 50 ("milliseconds to wait")) -> (s? t:f=w376:u32)
    n254 = Wait (ms)(milliseconds to wait=w376) -> ()  [unwired: 1 out]
  }
  n255 = while {
    shift-right: [w458] -> _
    shift-left: w5 -> [w458]
    stop <- w451 stop-if-true
    # "Stop loop if LED comms lost\nThis prevents excessive driver station\nerrors"
    # "LED Control"
    n256 = call "time_delta.vi"() -> ("dt (s)"=w456:dbl)  [unwired: 1 in]
    n257 = Reciprocal(x=w456) -> (1/x=→"LED Loop Rate (Hz)":dbl)
    n258 = call "LEDComms.vi"() -> ("error out"=w455:errorcluster)  [unwired: 11 in]
    n259 = Unbundle By Name(w455) -> ("status"=w454:bool)
    n260 = First Call?() -> (First Call?: T/F=w453:bool)
    n261 = call "Timed_DeBounce.vi"("Input"=w454, "Reset"=w453, "Hold Time(ms)"=u32 2000) -> ("Output"=w451:bool)
    n262 = Wait (ms)(milliseconds to wait=u32 50) -> ()  [unwired: 1 out]
  }
